vi "Imaging_Proc.vi"(5 "BioMAP file path":path=path "", 7 "Params.":variant, 8 "error in (no error)":errorcluster, 9 "Dynamic Params queue":refnum<queue>, 10 "Quit_UserEvent":refnum<user-event>, 11 "ControlQueueRef":variant) -> (0 "error out":errorcluster, 2 "Output":variant)   [LabVIEW 2013]
uses:
  Apps_static/ScanParams_SingleLine.ctl
  Files/BinaryHeader.ctl
  ControlDef/QueueRefs.ctl
  ControlDef/LaserCtrl_Method.ctl
  ControlDef/States-AToF.ctl
  <instrlib>/AnalogDiscSDKLv/VIs/DWF_CtrlQueue.ctl
  <instrlib>/AnalogDiscSDKLv/VIs/DWF_State.ctl
  <instrlib>/ESP300/Public/Data/ESP300_State.ctl
  <instrlib>/DG535/Command/DG535_States.ctl
  Hardware/BNC(QuantumComposers)/BNC_States.ctl
  Hardware/FemtoLaser(Legacy)/Laser_Status.ctl
  Hardware/DAQmx(Legacy)/DAQmx_Status.ctl
  ControlDef/Signal.ctl
  ProcessMethods/SignalAverager/ProcessStates.ctl
  Files/WriterState.ctl
  Files/Signal_Segment.ctl
  ControlDef/ProcessingMode.ctl
  Hardware/EPM2000(Legacy)/EPM2K_Status.ctl
  <instrlib>/AnalogDiscSDKLv/VIs/DWF_Signal.ctl
  ControlDef/SampleRateSelector.ctl
  DirectImaging_State.ctl
  Imaging_Params.ctl
  ProcessMethods/BioMapConversion/BioMAPWriterCoreParams.ctl
  ProcessMethods/Binning/BinType.ctl
  <vilib>/Utility/error.llb/DialogType.ctl
  <vilib>/Utility/miscctls.llb/LVRowAndColumnTypeDef.ctl
  <vilib>/picture/picture.llb/imagedata.ctl
  <userlib>/_OpenG.lib/comparison/comparison.llb/I32 Changed__ogtk.vi
  <vilib>/regexp/Match Regular Expression.xnode
  <instrlib>/ESP300/ESP300.lvlib
  <instrlib>/DG535/SRS_DG535_Lib.lvlib
  <userlib>/Utility/ErrorLog_lib.lvlib
  <instrlib>/AnalogDiscSDKLv/AnalogDiscSDKLv.lvlib
panel:
  out "POI diag.":cluster{"m/z":dbl, "Width(+/-)":dbl}[](array[cluster])
  in  "Contrast":cluster{dbl, dbl}(slide)={0.0, 255.0} scale=0.0..255.0
  in  "MaxiMass":dbl=300.0 format="%#_13g"
  in  "EnableBinning":bool
  out "Information":string
  in  "AutoScaleZ":bool
  in  "SaveImage":bool
  in  "Color Scheme":T1(ring)=enum."Rainbow"
  out "#SOL":i32
  out "#EOL":i32
  out "remaining lines":i32
  out "State":T2(ring)
  out "Line#":i32
  in  "Cancel":bool
  in  "Close/Quit":bool
  in  "Peaks of Interest":string[][](table)=[["300", "300"], ["58", ".45"], ["92", ".45"], ["114", ".45"]]
  in  "conv. coeff.":sgl=6553.0
  out "# average":i32
  in  "Start":bool
  out "ImagePreview":dbl[][](graph)
  in  "PeakOI #":i32 min=0 step=1
  out "MS (Raw)":cluster{"m/z_Array":dbl[], sgl[]}(graph)
  out "Iteration":i32
  out "Export File Path":path caption="Filename"
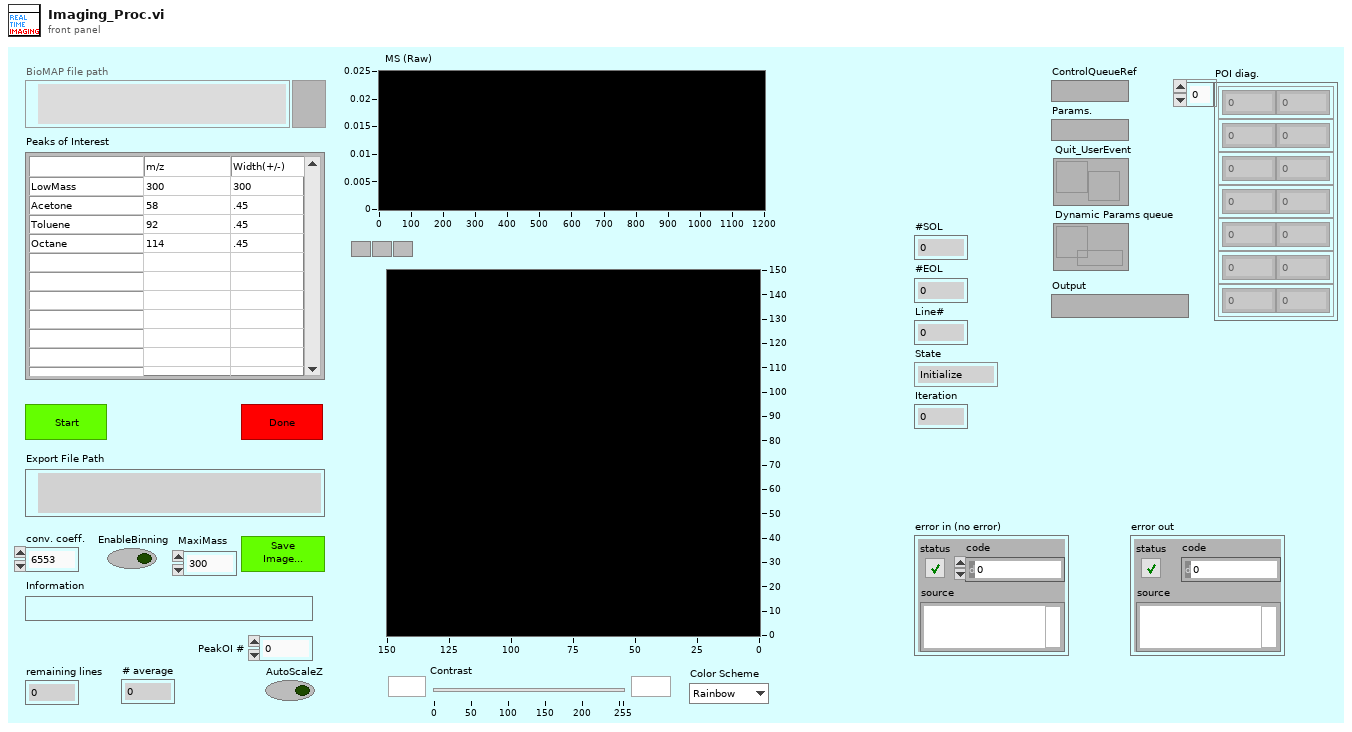
[diagram p1: front panel]
types:
  T1 = enum16{"Greyscale", "Rainbow", "Jet", "Rainbow_Wh", "Banded", "Seis", "InvertSeis", "Jaisnd", "TBD1"}
  T2 = enum16{"Initialize", "Open", "PrepScanParams", "WaitData", "Flush", "ScanResult", "CheckEndCondition", "Close", "Quit", "Refresh_Image", "Refresh_Profile", "Refresh_Spectra", "Refresh_RawSpectrum", "SaveMiddleFile", "Save_Image", "SetPeakOI"}
  T3 = cluster{"image path":path, "file refnum":refnum<file>}
  T4 = enum8{"Enabled", "Disabled", "Disabled and Grayed Out"}
  T5 = typedef "QueueRefs.ctl" = cluster{"LaserCtrlMethod":T6, "Apps":refnum<queue>, "MainDAQCoreQueue":refnum<queue>, "Micos":refnum<queue>, "ESP300":refnum<queue>, "SMC100":refnum<queue>, "SRS DG535":refnum<queue>, "BNC":refnum<queue>, "SDG_ii":refnum<queue>, "NI-USB_DAQmx":refnum<queue>, "ProcCore_CtrlQueue":refnum<queue>, "WriterCtrl":refnum<queue>, "WriterSIG":refnum<queue>, "Feedback":refnum<queue>, "EPM2000":refnum<queue>, "InfoRef":refnum<vi>, "AppsLock":T7, "ProcCore_SignalQueue":refnum<queue>}
  T6 = typedef "LaserCtrl_Method.ctl" = enum16{"SRS_DG535", "BNC", "SDG_II"}
  T7 = typedef "Semaphore RefNum" = refnum<k1>
  T8 = typedef "ProcessStates.ctl" = enum16{"Initialize", "Normal", "Display", "Write2Buffer", "CalcMzArray", "StartSave", "StopSave", "ConfigChanged", "EndOfLine", "SetFilterParams", "SetGraphsEnable", "SetAcquisitionParams", "ChangeDisplayIncrement", "ChangeRepRate", "SetWriterRef", "Quit", "StartOfLine"}
  T9 = cluster{"Average":i32, "X (Img)":i32, "Y (Img)":i32, "Spectra":sgl[]}
  T10 = typedef "BioMAPWriterCoreParams.ctl" = cluster{"File Header":T11, "mzCali.":dbl[], "m/z_Array":dbl[], "SampleRate":T12, "TrigDelay":dbl, "file refnum":refnum<file>, "file path":path, "PeakOI":cluster{"m/z":dbl, "Width(+/-)":dbl}[], "Binning":cluster{"Enable":bool, "BinType":T13, "BinWidth":dbl, "Maximum":dbl, "Minimum":dbl}}
  T11 = typedef "BinaryHeader.ctl" = cluster{"Start Position":dbl[], "StepWidth":dbl[], "Dimension":i32[], "SpecLength":i32}
  T12 = typedef "SampleRateSelector.ctl" = dbl
  T13 = typedef "BinType.ctl" = enum16{"ByTime", "ByScreen", "ByMass", "ToUnitMass"}
  T14 = typedef "Imaging_Params.ctl" = cluster{"File Header":T11, "ScanSpeed":dbl, "HighSpeed":dbl, "SampleRate":T12, "Rep.Rate (Hz)":dbl, "TrigDelay":dbl, "mzCali":dbl[], "KeepStill(ms)":u32, "SaveRaw":bool}
  T15 = typedef "DirectImaging_State.ctl" = cluster{"State":enum16{"Initialize", "Open", "PrepScanParams", "WaitData", "Flush", "ScanResult", "CheckEndCondition", "Close", "Quit", "Refresh_Image", "Refresh_Profile", "Refresh_Spectra", "Refresh_RawSpectrum", "SaveMiddleFile", "Save_Image", "SetPeakOI"}, "Para.":variant}
  T16 = cluster{"Save?":bool, "File Header":T11, "Scan#":i32, "ControlRefs":T5, "HighSpeed":dbl, "ScanSpeed":dbl, "SampleRate":T12, "mzCali.":dbl[], "TrigDelay":dbl, "InfoBarRef.":refnum<vi>}
  T17 = typedef "LVRowAndColumnTypeDef.ctl" = cluster{"Row":i32, "Column":i32}
  T18 = typedef "DialogType.ctl" = u16
  T19 = enum16{"open", "replace", "create", "open or create", "replace or create", "replace or create with confirmation"}
  T20 = cluster{"queue out":refnum<queue>, "queue out":refnum<queue>}
  T21 = typedef "Signal.ctl" = cluster{"Command":T8, "Params":variant}
  T22 = typedef "Signal_Segment.ctl" = cluster{"SampleRate":dbl, "TrigDelay":dbl, "SpecLength":dbl, "DAQ_Range":dbl, "Average#":i32, "Position":dbl[], "Spectrum":sgl[], "Calibr.":dbl[], "Pressure":dbl, "Desp_LaserEnergy":dbl, "PI_LaserEnergy":dbl, "Voltages Table":sgl[][], "ProcMode":T23, "Threshold":dbl, "Comment":string, "TickCount":dbl, "Time Stamp":timestamp}
  T23 = typedef "ProcessingMode.ctl" = enum16{"None", "Drop by Threshold", "TDC Simulate", "SetFilter"}
  T24 = typedef "ScanParams_SingleLine.ctl" = cluster{"Line Start":dbl[], "Line End":dbl[], "HighSpeed":dbl, "ScanSpeed":dbl, "KeepStill(ms)":u32, "InstruParams":dbl[]}
  T25 = typedef "imagedata.ctl" = cluster{"image type":i32, "image depth":i32, "image":u8[], "mask":u8[], "colors":u32[], "Rectangle":cluster{"left":i16, "top":i16, "right":i16, "bottom":i16}}
  T26 = cluster{"Rows Per Strip":i32, "Photometric":i32, "Compression Type":i32}
  T27 = typedef "IMAQ Image.ctl" = refnum<image>
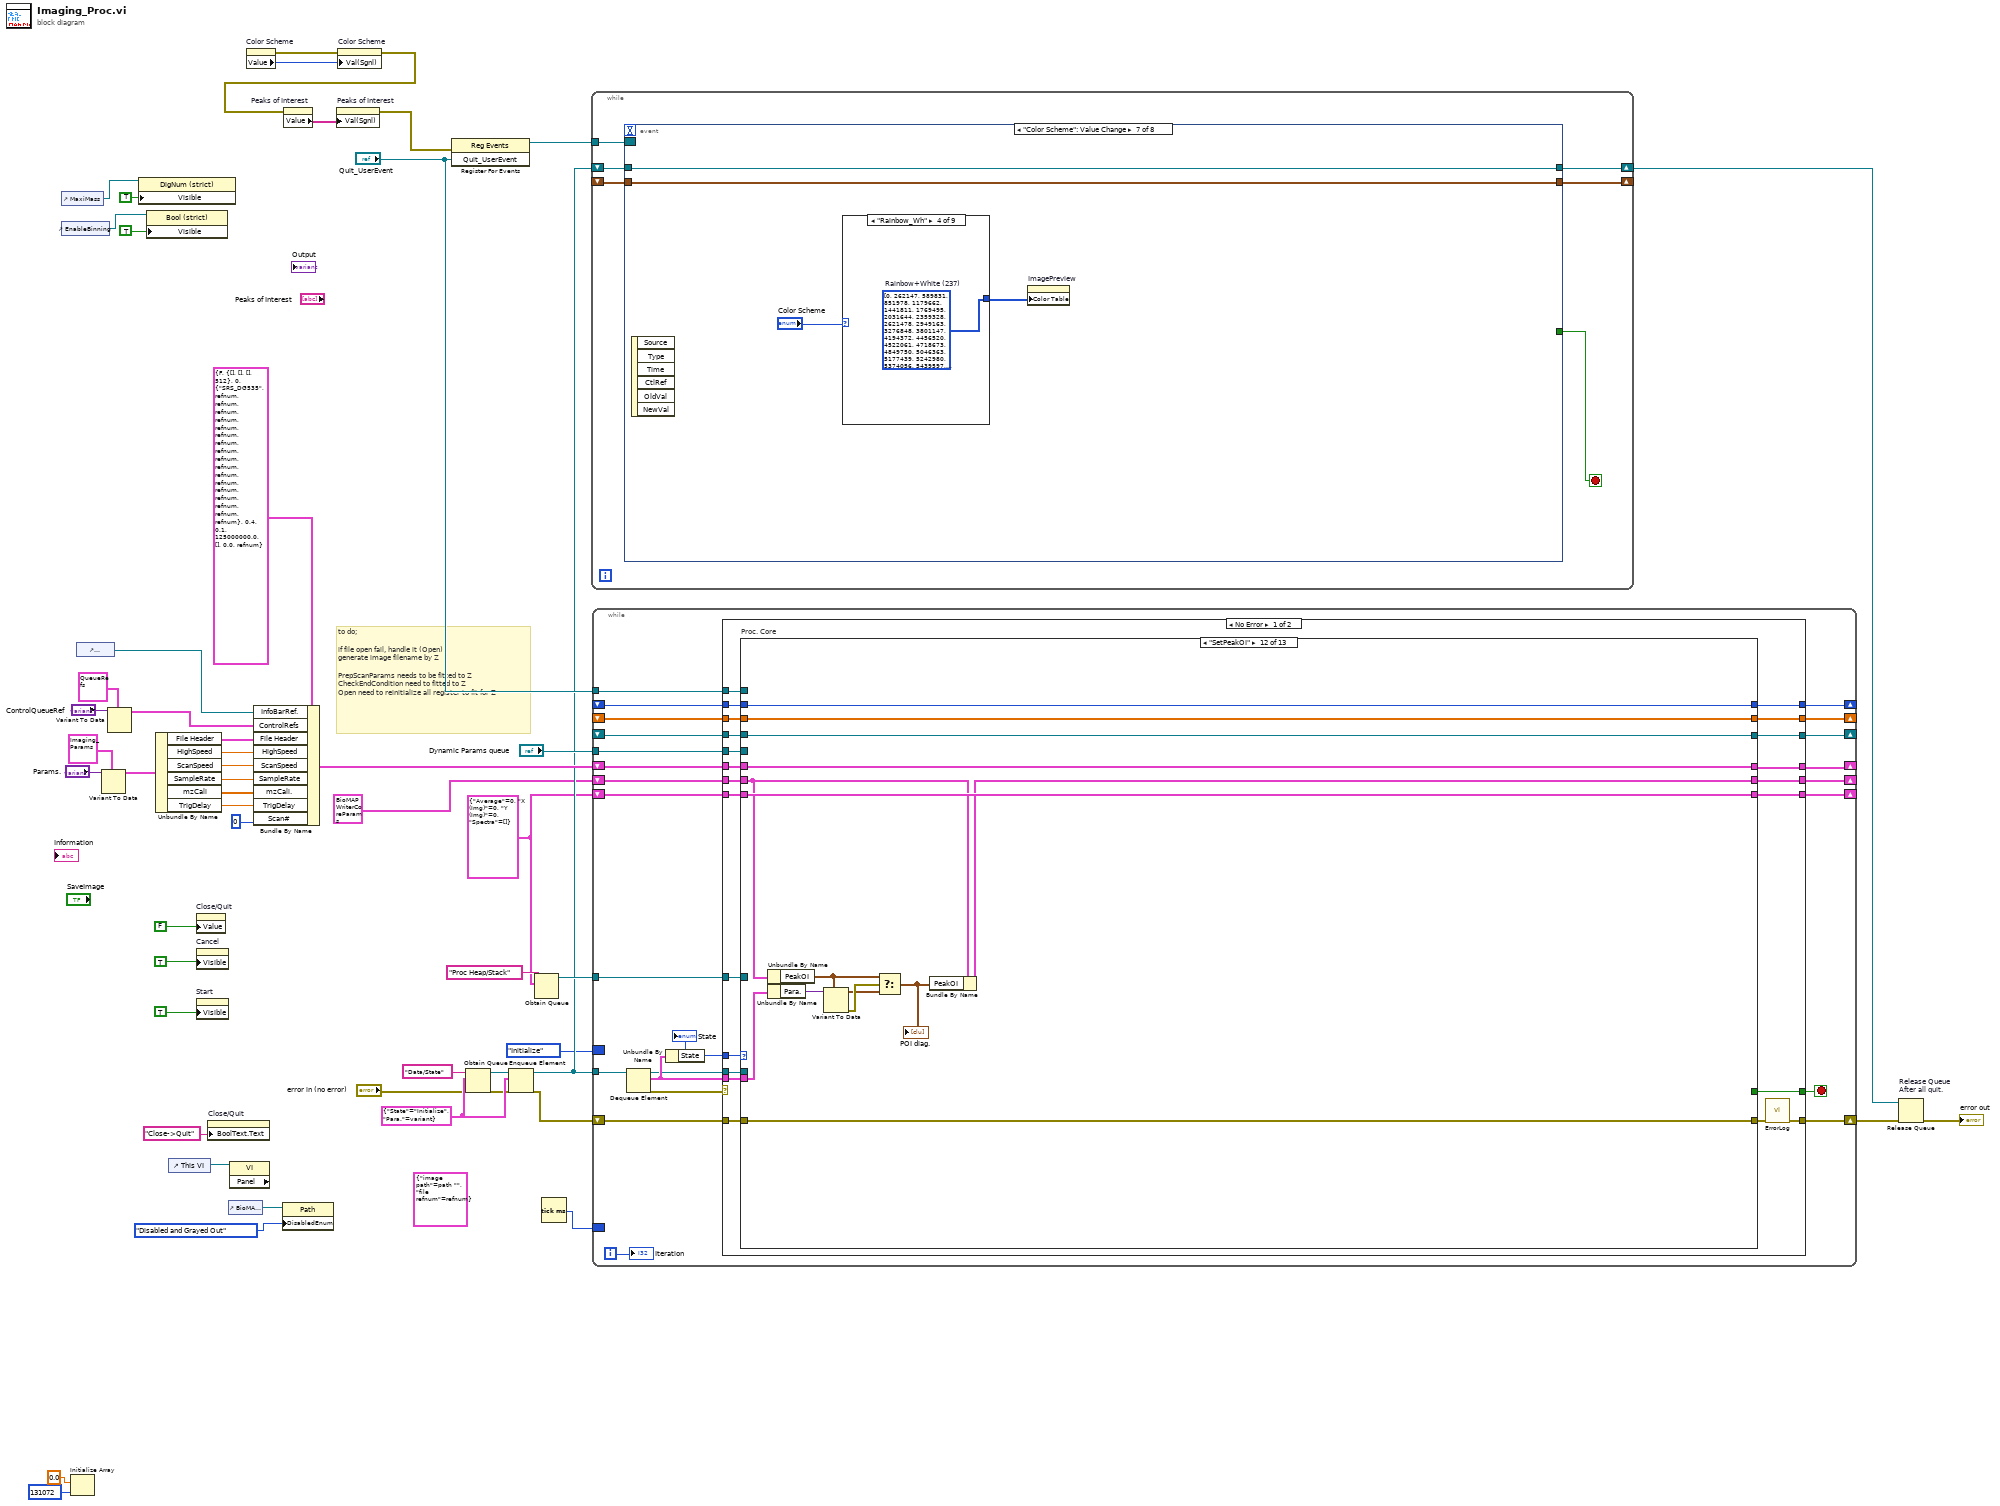
[diagram p0: block diagram]
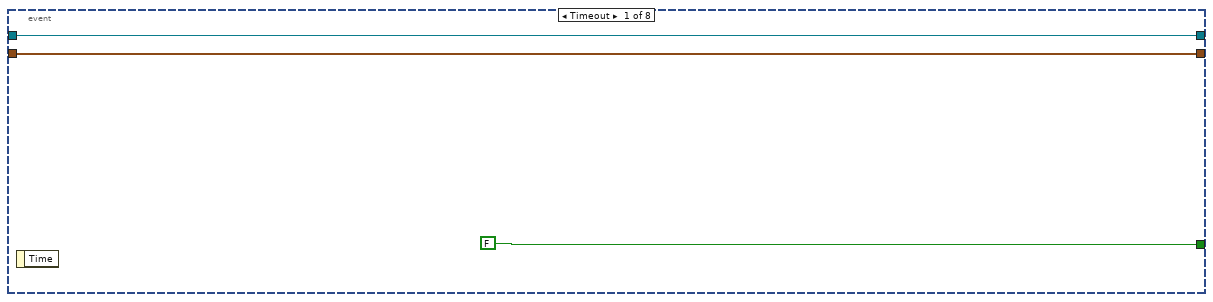
[diagram p2: hidden frame]
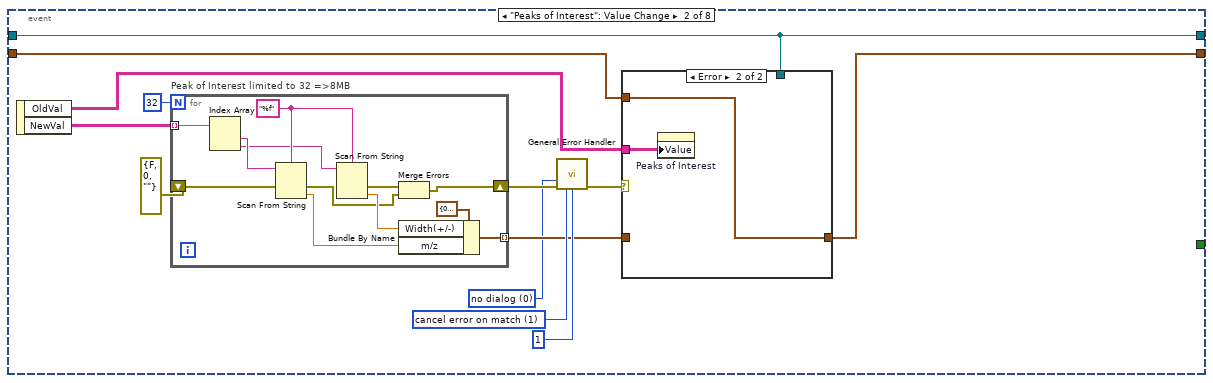
[diagram p3: hidden frame]
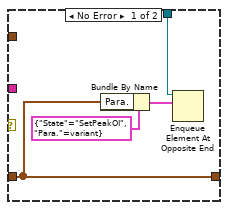
[diagram p4: hidden frame]
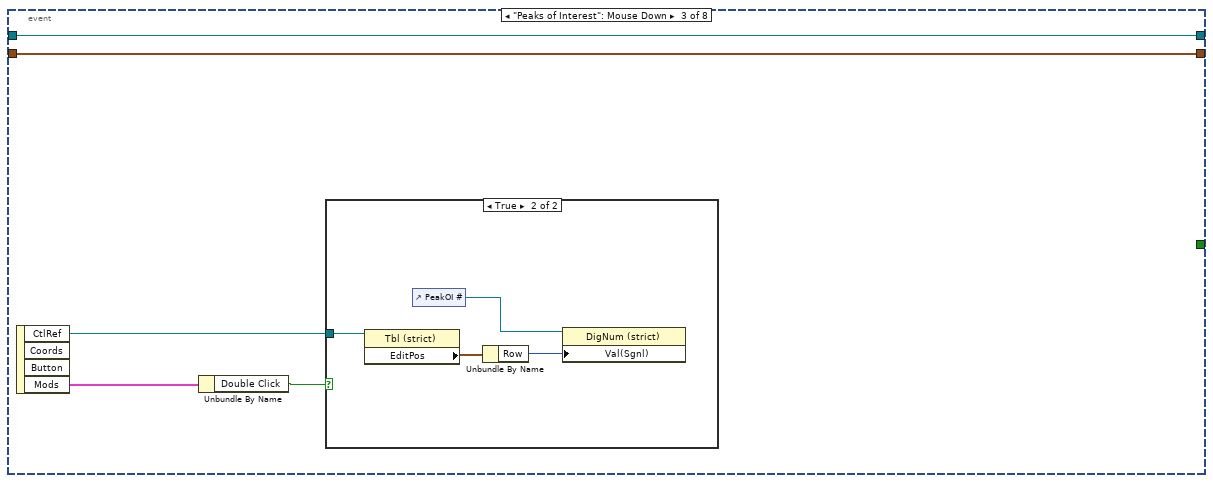
[diagram p5: hidden frame]
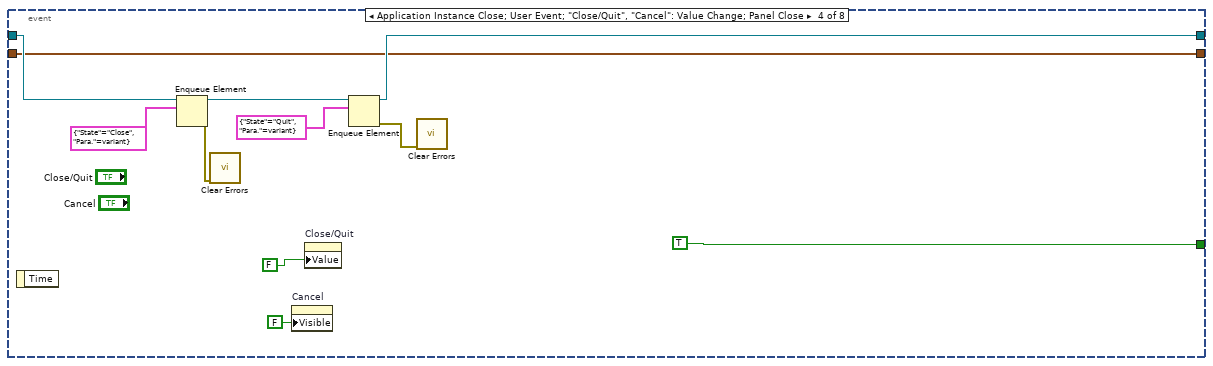
[diagram p7: hidden frame]
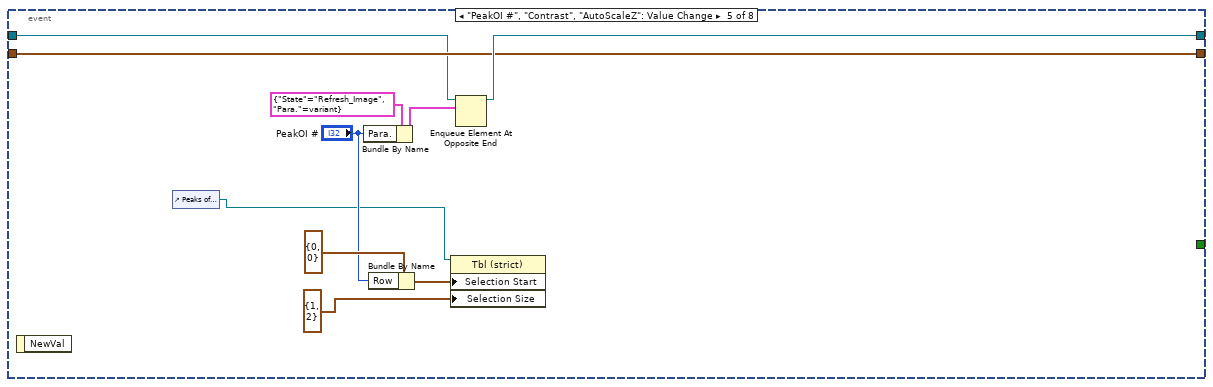
[diagram p8: hidden frame]
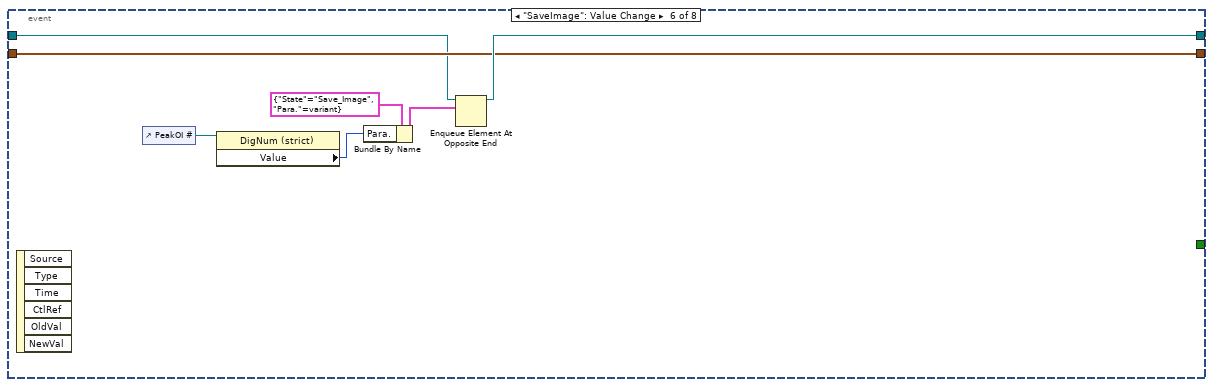
[diagram p9: hidden frame]
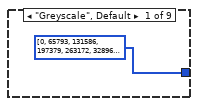
[diagram p10: hidden frame]
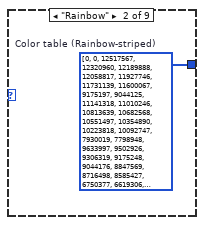
[diagram p11: hidden frame]
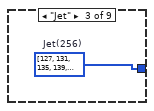
[diagram p12: hidden frame]
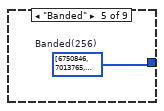
[diagram p13: hidden frame]
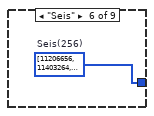
[diagram p14: hidden frame]
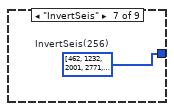
[diagram p15: hidden frame]
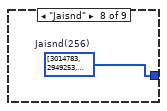
[diagram p16: hidden frame]
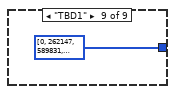
[diagram p17: hidden frame]
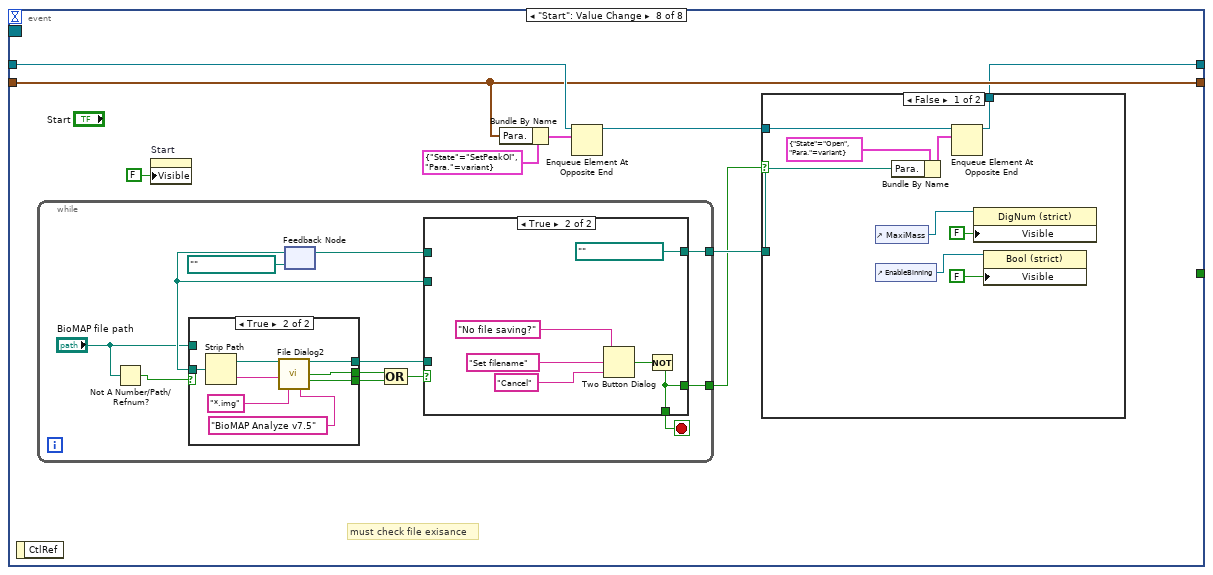
[diagram p18: hidden frame]
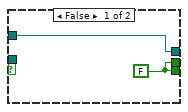
[diagram p20: hidden frame]
diagram:
  (unwired) T3 {"image path"=path "", "file refnum"=refnum} ("output cluster")
  w31 = T9 {"Average"=0, "X (Img)"=0, "Y (Img)"=0, "Spectra"=[]} ("output cluster")
  w43 = T15 {"State"=enum."Initialize", "Para."=variant}
  # "to do;\n\nif file open fail, handle it (Open)\ngenerate image filename by Z\n\nPrepScanParams needs to be fitted to Z\nCheckEndCondition need to fitted to Z\nOpen need to reinitialize all register to fit for Z"
  n1 = control-ref of="MaxiMass"() -> (w4:refnum<vi>)
  n2 = control-ref of="EnableBinning"() -> (w1:refnum<vi>)
  n3 = Initialize Array(sgl 0.0 ("element"), 131072 ("dimension size")) -> ()  [unwired: 1 out]
  n4 = control-ref of="Information"() -> (w10:refnum<vi>)
  n5 = Variant To Data(type=T14 {"File Header"={"Start Position"=[], "StepWidth"=[], "Dimension"=[], "SpecLength"=0}, "ScanSpeed"=0.0, "HighSpeed"=0.0, "SampleRate"=0.0, "Rep.Rate (Hz)"=0.0, "TrigDelay"=0.0, "mzCali"=[], "KeepStill(ms)"=0, "SaveRaw"=FALSE} ("BeamProfiling_Params"), Variant="Params.") -> (data=w38:T14)  [unwired: 1 in, 1 out]
  n6 = Variant To Data(type=T5 {"LaserCtrlMethod"=enum."SRS_DG535", "Apps"=refnum, "MainDAQCoreQueue"=refnum, "Micos"=refnum, "ESP300"=refnum, "SMC100"=refnum, "SRS DG535"=refnum, "BNC"=refnum, "SDG_ii"=refnum, "NI-USB_DAQmx"=refnum, "ProcCore_CtrlQueue"=refnum, "WriterCtrl"=refnum, "WriterSIG"=refnum, "Feedback"=refnum, "EPM2000"=refnum, "InfoRef"=refnum, "AppsLock"=refnum, "ProcCore_SignalQueue"=refnum} ("ControlRefs"), Variant="ControlQueueRef") -> (data=w18:T5)  [unwired: 1 in, 1 out]
  n7 = property class="DigNum (strict)"(reference=w4, "Visible"=TRUE) -> ()  [unwired: 1 in, 2 out]
  n8 = property class="Bool (strict)"(reference=w1, "Visible"=TRUE) -> ()  [unwired: 1 in, 2 out]
  n9 = Unbundle By Name(w38) -> ("File Header"=w37:T11, "HighSpeed"=w36:dbl, "ScanSpeed"=w35:dbl, "SampleRate"=w33:T12, "mzCali"=w24:dbl[], "TrigDelay"=w23:dbl)
  n10 = control-ref of="This VI"() -> (w22:refnum<vi>)
  n11 = property on="Close/Quit" class="Bool (strict)"("Value"=FALSE) -> ()  [unwired: 2 in, 2 out]
  n12 = property on="Cancel" class="Bool"("Visible"=TRUE) -> ()  [unwired: 2 in, 2 out]
  n13 = property on="Start" class="Bool"("Visible"=TRUE) -> ()  [unwired: 2 in, 2 out]
  n14 = property on="Close/Quit" class="Bool (strict)"("BoolText.Text"="Close->Quit" ("Boolean Text.Text")) -> ()  [unwired: 2 in, 2 out]
  n15 = control-ref of="BioMAP file path"() -> (w17:refnum<vi>)
  n16 = property class="VI" props=["Panel"](reference=w22) -> ()  [unwired: 1 in, 3 out]
  n17 = property on="Color Scheme" class="Enum (strict)"() -> (error out=w7:errorcluster, "Value"=w8:T1)  [unwired: 2 in, 1 out]
  n18 = Bundle By Name(cluster=T16 {"Save?"=FALSE, "File Header"={"Start Position"=[], "StepWidth"=[], "Dimension"=[], "SpecLength"=512}, "Scan#"=0, "ControlRefs"={"LaserCtrlMethod"=enum."SRS_DG535", "Apps"=refnum, "MainDAQCoreQueue"=refnum, "Micos"=refnum, "ESP300"=refnum, "SMC100"=refnum, "SRS DG535"=refnum, "BNC"=refnum, "SDG_ii"=refnum, "NI-USB_DAQmx"=refnum, "ProcCore_CtrlQueue"=refnum, "WriterCtrl"=refnum, "WriterSIG"=refnum, "Feedback"=refnum, "EPM2000"=refnum, "InfoRef"=refnum, "AppsLock"=refnum, "ProcCore_SignalQueue"=refnum}, "HighSpeed"=0.4, "ScanSpeed"=0.1, "SampleRate"=125000000.0, "mzCali."=[], "TrigDelay"=0.0, "InfoBarRef."=refnum} ("output cluster"), "InfoBarRef."=w10, "ControlRefs"=w18, "File Header"=w37, "HighSpeed"=w36, "ScanSpeed"=w35, "SampleRate"=w33, "mzCali."=w24, "TrigDelay"=w23, "Scan#"=0) -> (w47:T16)
  n19 = property class="Path"(reference=w17, "DisabledEnum"=T4."Disabled and Grayed Out" ("Disabled")) -> ()  [unwired: 1 in, 2 out]
  n20 = property on="Color Scheme" class="Enum (strict)"(error in=w7, "Val(Sgnl)"=w8) -> (error out=w5:errorcluster)  [unwired: 1 in, 1 out]
  n21 = property on="Peaks of Interest" class="Tbl (strict)"(error in=w5) -> ("Value"=w12:string[][])  [unwired: 1 in, 2 out]
  n22 = property on="Peaks of Interest" class="Tbl (strict)"("Val(Sgnl)"=w12) -> (error out=w6:errorcluster)  [unwired: 2 in, 1 out]
  n23 = register-events(error in=w6, "Quit_UserEvent") -> (reference out=w48:refnum<event-registration>)  [unwired: 1 in, 1 out]
  n24 = Obtain Queue(name (unnamed)="Data/State", element data type=w43, error in (no error)="error in (no error)") -> (queue out=w44:refnum<queue>, error out=w42:errorcluster)  [unwired: 2 in, 1 out]
  n25 = Enqueue Element(queue=w44, element=w43, error in (no error)=w42) -> (queue out=w40:refnum<queue>, error out=w32:errorcluster)  [unwired: 1 in, 1 out]
  n26 = Obtain Queue(name (unnamed)="Proc Heap/Stack", element data type=w31) -> (queue out=w53:refnum<queue>)  [unwired: 3 in, 2 out]
  n27 = Tick Count (ms)() -> (millisecond timer value=w30:u32)
  n28 = while {
    tunnel: w48 -> [w57]
    shift-right: [w56] -> w25
    shift-left: w40 -> [w59]
    shift-right: [w55] -> _
    shift-left: _ -> [w54]
    stop <- w58 stop-if-true
    n29 = event shown="[6] \"Color Scheme\": Value Change" {
      selector: w57 -> [_ _ _ _ _ _ _ _]
      dyn-events: _ -> [_ _ _ _ _ _ _ _]
      timeout: _ -> [_ _ _ _ _ _ _ _]
      tunnel: w59 -> [w61 w63 w98 w110 w119 w126 w134 w152]
      tunnel: [FALSE _ _ TRUE _ _ _ _] -> w58
      tunnel: [w61 w63 w98 w106 w121 w128 w134 w147] -> w56
      tunnel: [w60 w68 w94 w105 w120 w127 w131 w149] -> w55
      tunnel: w54 -> [w60 w66 w94 w105 w120 w127 w131 w149]
      event Timeout {
        n30 = event-data() -> ()  [unwired: 1 in, 1 out]
      }
      event "Peaks of Interest": Value Change {
        w64 = T18 0 items=["no dialog", "OK message", "continue or stop message", "OK message + warnings", "continue/stop + warnings"] ("type of dialog (OK msg:1)")
        w69 = 1 items=["no exception", "cancel error on match", "set error on match"] ("[exception action] (none:0)")
        n31 = event-data() -> ("OldVal"=w74:string[][], "NewVal"=w75:string[][])  [unwired: 1 in]
        n32 = for "Peak of Interest limited to 32 =>8MB" {
          N: 32 -> [_]
          tunnel: w75 -> [w87] mode=indexing
          shift-right: [w79] -> w70
          shift-left: errorcluster {"status"=FALSE, "code"=0, "source"=""} ("error IO") -> [w81]
          tunnel: [w80] -> w67 mode=indexing
          w86 = "%f" ("format string")
          n33 = Index Array(array=w87) -> (element #1=w77:string, element #2=w76:string)  [unwired: 2 in]
          n34 = Scan From String(format string=w86, input string=w77, error in=w81) -> (error out=w78:errorcluster, output 1=w83:dbl)  [unwired: 2 in, 2 out]
          n35 = Scan From String(format string=w86, input string=w76) -> (error out=w82:errorcluster, output 1=w84:dbl)  [unwired: 3 in, 2 out]
          n36 = Merge Errors(w82, w78) -> (w79:errorcluster)
          n37 = Bundle By Name(cluster=cluster{"m/z":dbl, "Width(+/-)":dbl} {"m/z"=0.0, "Width(+/-)"=0.0} ("Peak-Of-Interest"), "Width(+/-)"=w84, "m/z"=w83) -> (w80:cluster{"m/z":dbl, "Width(+/-)":dbl})
        }
        n38 = call <vilib>:"General Error Handler.vi"("type of dialog (OK msg:1)"=w64, "error in (no error)"=w70, "[exception action] (none:0)"=w69, "[exception code]"=1) -> ("error out"=w71:errorcluster)  [unwired: 7 in, 4 out]
        n39 = case shown="Error" w71 {
          tunnel: w74 -> [_ w93]
          tunnel: [w89 w92] -> w68
          tunnel: w67 -> [w89 _]
          tunnel: w66 -> [_ w92]
          tunnel: w63 -> [w88 _]
          frame No Error {
            n40 = Bundle By Name(cluster=T15 {"State"=enum."SetPeakOI", "Para."=variant} ("element"), "Para."=w89) -> (w90:T15)
            n41 = Enqueue Element At Opposite End(queue=w88, element=w90) -> ()  [unwired: 2 in, 3 out]
          }
          frame Error {
            n42 = property on="Peaks of Interest" class="Tbl (strict)"("Value"=w93) -> ()  [unwired: 2 in, 2 out]
          }
        }
      }
      event "Peaks of Interest": Mouse Down {
        n43 = event-data() -> ("CtlRef"=w95:refnum<vi>, "Mods"=w96:cluster{"Double Click":bool, "Menu Key":bool})  [unwired: 1 in, 2 out]
        n44 = Unbundle By Name(w96) -> ("Double Click"=w97:bool)
        n45 = case shown="True" w97 {
          tunnel: w95 -> [_ w101]
          frame False {
          }
          frame True {
            n46 = property class="Tbl (strict)"(reference=w101) -> ("EditPos"=w102:T17)  [unwired: 1 in, 2 out]
            n47 = control-ref of="PeakOI #"() -> (w99:refnum<vi>)
            n48 = Unbundle By Name(w102) -> ("Row"=w100:i32)
            n49 = property class="DigNum (strict)"(reference=w99, "Val(Sgnl)"=w100) -> ()  [unwired: 1 in, 2 out]
          }
        }
      }
      event Application Instance Close; User Event; "Close/Quit", "Cancel": Value Change; Panel Close {
        n50 = event-data() -> ()  [unwired: 1 in, 1 out]
        n51 = Enqueue Element(queue=w110, element=T15 {"State"=enum."Close", "Para."=variant}) -> (queue out=w111:refnum<queue>, error out=w109:errorcluster)  [unwired: 2 in, 1 out]
        n52 = call <vilib>:"Clear Errors.vi"("error in (no error)"=w109) -> ()  [unwired: 6 in, 1 out]
        n53 = property on="Cancel" class="Bool"("Visible"=FALSE) -> ()  [unwired: 2 in, 2 out]
        n54 = property on="Close/Quit" class="Bool (strict)"("Value"=FALSE) -> ()  [unwired: 2 in, 2 out]
        n55 = Enqueue Element(queue=w111, element=T15 {"State"=enum."Quit", "Para."=variant}) -> (queue out=w106:refnum<queue>, error out=w112:errorcluster)  [unwired: 2 in, 1 out]
        n56 = call <vilib>:"Clear Errors.vi"("error in (no error)"=w112) -> ()  [unwired: 6 in, 1 out]
      }
      event "PeakOI #", "Contrast", "AutoScaleZ": Value Change {
        n57 = event-data() -> ()  [unwired: 1 in, 1 out]
        n58 = control-ref of="Peaks of Interest"() -> (w114:refnum<vi>)
        n59 = Bundle By Name(cluster=T15 {"State"=enum."Refresh_Image", "Para."=variant} ("element"), "Para."="PeakOI #") -> (w122:T15)
        n60 = Bundle By Name(cluster=T17 {"Row"=0, "Column"=0} ("Selection Start"), "Row"="PeakOI #") -> (w117:T17)
        n61 = property on="Property Node" class="Tbl (strict)"(reference=w114, "Selection Start"=w117, "Selection Size"=T17 {"Row"=1, "Column"=2}) -> ()  [unwired: 1 in, 2 out]
        n62 = Enqueue Element At Opposite End(queue=w119, element=w122) -> (queue out=w121:refnum<queue>)  [unwired: 2 in, 2 out]
      }
      event "SaveImage": Value Change {
        n63 = event-data() -> ()  [unwired: 1 in, 6 out]
        n64 = control-ref of="PeakOI #"() -> (w125:refnum<vi>)
        n65 = property class="DigNum (strict)"(reference=w125) -> ("Value"=w124:i32)  [unwired: 1 in, 2 out]
        n66 = Bundle By Name(cluster=T15 {"State"=enum."Save_Image", "Para."=variant} ("element"), "Para."=w124) -> (w129:T15)
        n67 = Enqueue Element At Opposite End(queue=w126, element=w129) -> (queue out=w128:refnum<queue>)  [unwired: 2 in, 2 out]
      }
      event "Color Scheme": Value Change {
        n68 = event-data() -> ()  [unwired: 1 in, 6 out]
        n69 = case shown="\"Rainbow_Wh\"" "Color Scheme" {
          tunnel: [u32[] [0, 65793, 131586, 197379, 263172, 328965, 394758, 460551, 526344, 592137, 657930, 723723, 789516, 855309, 921102, 986895, 1052688, 1118481, 1184274, 1250067, 1315860, 1381653, 1447446, 1513239, 1579032, 1644825, 1710618, 1776411, 1842204, 1907997, 1973790, 2039583, 2105376, 2171169, 2236962, 2302755, 2368548, 2434341, 2500134, 2565927, 2631720, 2697513, 2763306, 2829099, 2894892, 2960685, 3026478, 3092271, 3158064, 3223857, 3289650, 3355443, 3421236, 3487029, 3552822, 3618615, 3684408, 3750201, 3815994, 3881787, 3947580, 4013373, 4079166, 4144959, 4210752, 4276545, 4342338, 4408131, 4473924, 4539717, 4605510, 4671303, 4737096, 4802889, 4868682, 4934475, 5000268, 5066061, 5131854, 5197647, 5263440, 5329233, 5395026, 5460819, 5526612, 5592405, 5658198, 5723991, 5789784, 5855577, 5921370, 5987163, 6052956, 6118749, 6184542, 6250335, 6316128, 6381921, 6447714, 6513507, 6579300, 6645093, 6710886, 6776679, 6842472, 6908265, 6974058, 7039851, 7105644, 7171437, 7237230, 7303023, 7368816, 7434609, 7500402, 7566195, 7631988, 7697781, 7763574, 7829367, 7895160, 7960953, 8026746, 8092539, 8158332, 8224125, 8289918, 8355711, 8421504, 8487297, 8553090, 8618883, 8684676, 8750469, 8816262, 8882055, 8947848, 9013641, 9079434, 9145227, 9211020, 9276813, 9342606, 9408399, 9474192, 9539985, 9605778, 9671571, 9737364, 9803157, 9868950, 9934743, 10000536, 10066329, 10132122, 10197915, 10263708, 10329501, 10395294, 10461087, 10526880, 10592673, 10658466, 10724259, 10790052, 10855845, 10921638, 10987431, 11053224, 11119017, 11184810, 11250603, 11316396, 11382189, 11447982, 11513775, 11579568, 11645361, 11711154, 11776947, 11842740, 11908533, 11974326, 12040119, 12105912, 12171705, 12237498, 12303291, 12369084, 12434877, 12500670, 12566463, 12632256, 12698049, 12763842, 12829635, 12895428, 12961221, 13027014, 13092807, 13158600, 13224393, 13290186, 13355979, 13421772, 13487565, 13553358, 13619151, 13684944, 13750737, 13816530, 13882323, 13948116, 14013909, 14079702, 14145495, 14211288, 14277081, 14342874, 14408667, 14474460, 14540253, 14606046, 14671839, 14737632, 14803425, 14869218, 14935011, 15000804, 15066597, 15132390, 15198183, 15263976, 15329769, 15395562, 15461355, 15527148, 15592941, 15658734, 15724527, 15790320, 15856113, 15921906, 15987699, 16053492, 16119285, 16185078, 16250871, 16316664, 16382457, 16448250, 16514043, 16579836, 16645629, 16711422, 16777215] ("Array") w136 w137 w138 w139 w140 w141 w142 u32[] [0, 262147, 589831, 851978, 1179662, 1441811, 1769495, 2031644, 2359328, 2621478, 2949163, 3276848, 3801147, 4194372, 4456520, 4522061, 4718673, 4849750, 5046363, 5177439, 5242980, 5374056, 5439597, 5505142, 5636218, 5767300, 5636232, 5701773, 5701777, 5701782, 5570714, 5505183, 5505187, 5505192, 5177521, 5111990, 5046458, 4980927, 4587720, 4456652, 4325585, 3932374, 3801306, 3604703, 3014888, 2818284, 2621681, 2359541, 2162938, 1638655, 1048831, 786687, 262399, 255, 1279, 4351, 5631, 6655, 7679, 9983, 11007, 12031, 13311, 16383, 17407, 18687, 21759, 23039, 24063, 25087, 27391, 28415, 29439, 30719, 32767, 34815, 36095, 39167, 40447, 41471, 42495, 44799, 45823, 46847, 48127, 50175, 51199, 55551, 56575, 57855, 58879, 59903, 62207, 63231, 64255, 65535, 65526, 65522, 65518, 65505, 65496, 65492, 65483, 65479, 65475, 65471, 65467, 65458, 65454, 65450, 65437, 65432, 65424, 65415, 65411, 65407, 65403, 65394, 65390, 65386, 65382, 65369, 65364, 65360, 65356, 65343, 65339, 65335, 65326, 65322, 65318, 65305, 65301, 65296, 65292, 65288, 65280, 589568, 851712, 1441536, 1703680, 1965824, 2817792, 3079936, 3407616, 3669760, 4194048, 4456192, 4783872, 5046016, 5897984, 6160128, 6422272, 7274240, 7536384, 7864064, 8126208, 8650496, 8912640, 9240320, 9502464, 10092288, 10616576, 10878720, 11730688, 11992832, 12320512, 12582656, 13106944, 13369088, 13696768, 13958912, 14548736, 14810880, 15924992, 16187136, 16449280, 16776960, 16775680, 16773632, 16772608, 16771328, 16770304, 16768256, 16766976, 16765952, 16762624, 16760576, 16759552, 16757248, 16756224, 16755200, 16753920, 16752896, 16750848, 16749568, 16748544, 16745216, 16744192, 16742144, 16739840, 16738816, 16737792, 16736512, 16734464, 16733440, 16732160, 16731136, 16727808, 16726784, 16725760, 16724736, 16721408, 16720384, 16719104, 16717056, 16716032, 16714752, 16711680, 16711680, 16711680, 16711680, 16711680, 16711680, 16711680, 16711680, 16711680, 16711680, 16711680, 16711680, 16711680, 16711680, 16711680, 16711680, 16711680, 16711680, 15527148, 15592941, 15658734, 15724527, 15790320, 15856113, 15921906, 15987699, 16053492, 16119285, 16185078, 16250871, 16316664, 16382457, 16448250, 16514043, 16579836, 16645629, 16711422, 16777215] ("appended array")] -> w132
          frame "Greyscale", Default {
          }
          frame "Rainbow" {
            w136 = u32[] [0, 0, 12517567, 12320960, 12189888, 12058817, 11927746, 11731139, 11600067, 9175197, 9044125, 11141318, 11010246, 10813639, 10682568, 10551497, 10354890, 10223818, 10092747, 7930019, 7798948, 9633997, 9502926, 9306319, 9175248, 9044176, 8847569, 8716498, 8585427, 6750377, 6619306, 8126677, 7995606, 7798999, 7667927, 7536856, 7340249, 7209178, 7078106, 5505199, 5374128, 6619357, 6488285, 6291678, 6160607, 6029536, 5832929, 5701857, 5570786, 4325557, 4194486, 5112036, 4980965, 4784358, 4653287, 4522215, 4325608, 4194537, 4063466, 3080380, 3014844, 3604716, 3408109, 3277038, 3277038, 3145966, 3014895, 2818288, 2687217, 2556145, 1900738, 1769666, 2097396, 1900789, 1769717, 1638646, 1507575, 1310968, 1179896, 1048825, 721096, 590024, 590075, 393468, 262397, 131326, 255, 1791, 3327, 4863, 5068, 6348, 9471, 11007, 12543, 14079, 15615, 17151, 18687, 20223, 17612, 18636, 25087, 26623, 28159, 29695, 31231, 32767, 34303, 35839, 29900, 31180, 40447, 41983, 43775, 45311, 46847, 48383, 49919, 51455, 42444, 43724, 56063, 57599, 59135, 60671, 62207, 63743, 65535, 65528, 52418, 52413, 65510, 65504, 65498, 65492, 65486, 65480, 65474, 65468, 52369, 52364, 65449, 65443, 65437, 65431, 65425, 65419, 65413, 65407, 52321, 52316, 65389, 65383, 65377, 65371, 65364, 65358, 65352, 65346, 52272, 52267, 65328, 65322, 65316, 65310, 65304, 65298, 65292, 65286, 52224, 314368, 851712, 1244928, 1638144, 2031360, 2424576, 2817792, 3211008, 3604224, 3197952, 3525632, 4783872, 5177088, 5635840, 6029056, 6422272, 6815488, 7208704, 7601920, 6409216, 6736896, 6736896, 8781568, 9174784, 9568000, 9961216, 10354432, 10747648, 11206400, 11599616, 9554944, 9882624, 12779264, 13172480, 13565696, 13958912, 14352128, 14745344, 15138560, 15531776, 12766208, 13093888, 16776960, 16775170, 16773637, 16771847, 16770314, 16768780, 16766991, 16765457, 13411088, 13409810, 16760601, 16758812, 16757278, 16755745, 16753955, 16752422, 16750888, 16749099, 13398052, 13396774, 16744243, 16742704, 16741166, 16739884, 16738345, 16736807, 16735269, 16733730, 13385753, 13384728, 16729371, 16727833, 16726295, 16725012, 16723474, 16721936, 16720397, 16718859, 13373959, 13372677, 16714500, 16712962, 16777215]  # Color table (Rainbow-striped)
          }
          frame "Jet" {
            w137 = u32[] [127, 131, 135, 139, 143, 147, 151, 155, 159, 163, 167, 171, 175, 179, 183, 187, 191, 195, 199, 203, 207, 211, 215, 219, 223, 227, 231, 235, 239, 243, 247, 251, 255, 1279, 2303, 3327, 4351, 5375, 6399, 7423, 8447, 9471, 10495, 11519, 12543, 13567, 14591, 15615, 16639, 17663, 18687, 19711, 20735, 21759, 22783, 23807, 24831, 25855, 26879, 27903, 28927, 29951, 30975, 31999, 33023, 34047, 35071, 36095, 37119, 38143, 39167, 40191, 41215, 42239, 43263, 44287, 45311, 46335, 47359, 48383, 49407, 50431, 51455, 52479, 53503, 54527, 55551, 56575, 57599, 58623, 59647, 60671, 61695, 62719, 63743, 64767, 131069, 393209, 655349, 917489, 1179629, 1441769, 1703909, 1966049, 2228189, 2490329, 2752469, 3014609, 3276749, 3538889, 3801029, 4063169, 4325309, 4587449, 4849589, 5111729, 5373869, 5636009, 5898149, 6160289, 6422429, 6684569, 6946709, 7208849, 7470989, 7733129, 7995269, 8257409, 8519549, 8781689, 9043829, 9305969, 9568109, 9830249, 10092389, 10354529, 10616669, 10878809, 11140949, 11403089, 11665229, 11927369, 12189509, 12451649, 12713789, 12975929, 13238069, 13500209, 13762349, 14024489, 14286629, 14548769, 14810909, 15073049, 15335189, 15597329, 15859469, 16121609, 16383749, 16645889, 16776192, 16775168, 16774144, 16773120, 16772096, 16771072, 16770048, 16769024, 16768000, 16766976, 16765952, 16764928, 16763904, 16762880, 16761856, 16760832, 16759808, 16758784, 16757760, 16756736, 16755712, 16754688, 16753664, 16752640, 16751616, 16750592, 16749568, 16748544, 16747520, 16746496, 16745472, 16744448, 16743424, 16742400, 16741376, 16740352, 16739328, 16738304, 16737280, 16736256, 16735232, 16734208, 16733184, 16732160, 16731136, 16730112, 16729088, 16728064, 16727040, 16726016, 16724992, 16723968, 16722944, 16721920, 16720896, 16719872, 16718848, 16717824, 16716800, 16715776, 16714752, 16713728, 16712704, 16711680, 16449536, 16187392, 15925248, 15663104, 15400960, 15138816, 14876672, 14614528, 14352384, 14090240, 13828096, 13565952, 13303808, 13041664, 12779520, 12517376, 12255232, 11993088, 11730944, 11468800, 11206656, 10944512, 10682368, 10420224, 10158080, 9895936, 9633792, 9371648, 9109504, 8847360, 8585216, 8323072]  # Jet(256)
          }
          frame "Rainbow_Wh" {
            w138 = u32[] [0, 262147, 589831, 851978, 1179662, 1441811, 1769495, 2031644, 2359328, 2621478, 2949163, 3276848, 3801147, 4194372, 4456520, 4522061, 4718673, 4849750, 5046363, 5177439, 5242980, 5374056, 5439597, 5505142, 5636218, 5767300, 5636232, 5701773, 5701777, 5701782, 5570714, 5505183, 5505187, 5505192, 5177521, 5111990, 5046458, 4980927, 4587720, 4456652, 4325585, 3932374, 3801306, 3604703, 3014888, 2818284, 2621681, 2359541, 2162938, 1638655, 1048831, 786687, 262399, 255, 1279, 4351, 5631, 6655, 7679, 9983, 11007, 12031, 13311, 16383, 17407, 18687, 21759, 23039, 24063, 25087, 27391, 28415, 29439, 30719, 32767, 34815, 36095, 39167, 40447, 41471, 42495, 44799, 45823, 46847, 48127, 50175, 51199, 55551, 56575, 57855, 58879, 59903, 62207, 63231, 64255, 65535, 65526, 65522, 65518, 65505, 65496, 65492, 65483, 65479, 65475, 65471, 65467, 65458, 65454, 65450, 65437, 65432, 65424, 65415, 65411, 65407, 65403, 65394, 65390, 65386, 65382, 65369, 65364, 65360, 65356, 65343, 65339, 65335, 65326, 65322, 65318, 65305, 65301, 65296, 65292, 65288, 65280, 589568, 851712, 1441536, 1703680, 1965824, 2817792, 3079936, 3407616, 3669760, 4194048, 4456192, 4783872, 5046016, 5897984, 6160128, 6422272, 7274240, 7536384, 7864064, 8126208, 8650496, 8912640, 9240320, 9502464, 10092288, 10616576, 10878720, 11730688, 11992832, 12320512, 12582656, 13106944, 13369088, 13696768, 13958912, 14548736, 14810880, 15924992, 16187136, 16449280, 16776960, 16775680, 16773632, 16772608, 16771328, 16770304, 16768256, 16766976, 16765952, 16762624, 16760576, 16759552, 16757248, 16756224, 16755200, 16753920, 16752896, 16750848, 16749568, 16748544, 16745216, 16744192, 16742144, 16739840, 16738816, 16737792, 16736512, 16734464, 16733440, 16732160, 16731136, 16727808, 16726784, 16725760, 16724736, 16721408, 16720384, 16719104, 16717056, 16716032, 16714752, 16711680, 16711680, 16711680, 16711680, 16711680, 16711680, 16711680, 16711680, 16711680, 16711680, 16711680, 16711680, 16711680, 16711680, 16711680, 16711680, 16711680, 16711680, 16777215, 16777215, 16777215, 16777215, 16777215, 16777215, 16777215, 16777215, 16777215, 16777215, 16777215, 16777215, 16777215, 16777215, 16777215, 16777215, 16777215, 16777215, 16777215, 16777215]  # Rainbow+White (237)
          }
          frame "Banded" {
            w139 = u32[] [6750846, 7013765, 7211659, 7409807, 7476371, 7411604, 7214997, 7017621, 6754453, 6490776, 6358685, 6226596, 6226092, 6226101, 6226109, 6227140, 6293961, 6296012, 6297806, 6233806, 5906635, 5512904, 4922053, 4199363, 3542212, 2950855, 2425550, 2031830, 1638622, 1376741, 1246954, 1314285, 1447407, 1975278, 2305771, 2372838, 2242272, 1783259, 1323992, 799448, 340956, 79842, 15849, 17905, 151543, 481786, 1009148, 1667324, 2193914, 2457333, 2523375, 2260968, 1801698, 1276895, 752607, 360418, 99816, 36335, 38390, 237307, 632574, 1158654, 1815550, 2275323, 2537717, 2471662, 2208487, 1683426, 1158879, 634847, 308451, 48362, 50673, 52728, 316924, 777214, 1302782, 1893373, 2352122, 2548212, 2481645, 2087398, 1628129, 1038303, 580576, 254949, 60394, 62189, 129520, 392688, 851694, 1441515, 2031078, 2423264, 2552791, 2419661, 2024898, 1499321, 974770, 516526, 190124, 60844, 62635, 129707, 458153, 982695, 1572516, 2161825, 2488475, 2552211, 2353800, 1893501, 1368177, 843623, 451166, 124759, 61010, 62797, 195401, 589383, 1113670, 1703494, 2227014, 2553410, 2551868, 2287665, 1827364, 1302294, 974603, 1040900, 1239041, 1699840, 2291200, 3013379, 3866121, 4783634, 5635611, 6355746, 6878502, 7073317, 7071521, 7004697, 6938385, 7069705, 7398403, 7858688, 8515840, 9172992, 9894916, 10550795, 11140627, 11599132, 11926051, 12055590, 11988261, 11855391, 11723032, 11788047, 11984904, 12510467, 13101824, 13759232, 14416129, 15006981, 15400460, 15728149, 15858974, 15857956, 15659558, 15395620, 15065886, 14736150, 14669582, 14800391, 15128322, 15587840, 16047616, 16441345, 16637958, 16703246, 16702743, 16570656, 16307237, 15846438, 15385379, 14924316, 14660116, 14658828, 14854661, 15182337, 15641344, 16100352, 16493826, 16690440, 16690192, 16690201, 16492833, 16163878, 15703078, 15242018, 14846235, 14647058, 14645003, 14840068, 15232513, 15690496, 16083200, 16410371, 16541193, 16541202, 16410139, 16213282, 15818789, 15292709, 14831136, 14434840, 14169616, 14166537, 14360579, 14686208, 15077888, 15404288, 15600132, 15665675, 15536665, 15342119, 15015986, 14558008, 14033211, 13507643, 13047097, 12848439, 12781367, 12911162, 13107263, 13303877, 13500748, 13501524, 13371996, 13177188, 12851050, 12393581, 11869549, 11278955, 10753384, 10293092, 9963875, 9765987, 9765220, 9764967, 9699434, 9634157, 9372526, 9111662, 8719469, 8261738]  # Banded(256)
          }
          frame "Seis" {
            w140 = u32[] [11206656, 11403264, 11599872, 11796480, 11993088, 12189696, 12386304, 12582912, 12779520, 12976128, 13172736, 13369344, 13565952, 13762560, 13959168, 14155776, 14352384, 14548992, 14745600, 14942208, 15138816, 15335424, 15532032, 15728640, 15925248, 16121856, 16318464, 16515072, 16711680, 16712448, 16713216, 16713984, 16714752, 16715520, 16716288, 16717056, 16717824, 16718592, 16719360, 16720128, 16720896, 16721664, 16722432, 16723200, 16723968, 16724736, 16725504, 16726272, 16727040, 16727808, 16728576, 16729344, 16730112, 16730880, 16731648, 16732416, 16733184, 16733952, 16734720, 16735488, 16736256, 16737024, 16737792, 16738560, 16739328, 16740096, 16740864, 16741632, 16742400, 16743168, 16743936, 16744448, 16745216, 16745984, 16746752, 16747520, 16748288, 16749056, 16749824, 16750592, 16751360, 16752128, 16752896, 16753664, 16754432, 16755200, 16755968, 16756736, 16757504, 16758272, 16759040, 16759808, 16760576, 16761344, 16762112, 16762880, 16763648, 16764416, 16765184, 16765952, 16766720, 16767488, 16768256, 16769024, 16769792, 16770560, 16771328, 16772096, 16772864, 16773632, 16774400, 16775168, 16775936, 16776704, 16776960, 16776960, 16776960, 16776960, 16776960, 16776960, 16776960, 16776960, 16776960, 16776960, 16776960, 16776960, 16776960, 16776960, 16776960, 16776960, 16776960, 16776960, 16776960, 16776960, 16776960, 16776960, 16776960, 16776960, 16776960, 16776960, 16776960, 16776960, 16645888, 16252673, 15924994, 15531779, 15138565, 14745350, 14352135, 14024456, 13631241, 13238026, 12844811, 12451596, 12123917, 11730702, 11337487, 10944272, 10551057, 10223378, 9830163, 9436948, 9043733, 8650518, 8322840, 7929625, 7536410, 7143195, 6749980, 6422301, 6029086, 5766944, 5570083, 5373222, 5176617, 4979756, 4717615, 4520753, 4324148, 4127287, 3930682, 3733821, 3471679, 3274818, 3078213, 2881352, 2684747, 2487886, 2225744, 2028883, 1832278, 1635417, 1438556, 1241950, 979553, 782948, 586087, 389482, 192620, 60784, 59509, 57979, 56704, 55173, 53642, 52367, 50836, 49305, 48030, 46499, 44968, 43694, 42163, 40888, 39357, 37826, 36551, 35020, 33489, 32214, 30684, 29409, 27878, 26347, 25072, 23541, 22010, 20735, 19965, 19195, 18426, 17912, 17142, 16372, 15603, 14833, 14319, 13549, 12780, 12010, 11240, 10726, 9957, 9187, 8417, 7647, 7134, 6364, 5594, 4824, 4055, 3541, 2771, 2001, 1232, 462]  # Seis(256)
          }
          frame "InvertSeis" {
            w141 = u32[] [462, 1232, 2001, 2771, 3541, 4055, 4824, 5594, 6364, 7134, 7647, 8417, 9187, 9957, 10726, 11240, 12010, 12780, 13549, 14319, 14833, 15603, 16372, 17142, 17912, 18426, 19195, 19965, 20735, 22010, 23541, 25072, 26347, 27878, 29409, 30684, 32214, 33489, 35020, 36551, 37826, 39357, 40888, 42163, 43694, 44968, 46499, 48030, 49305, 50836, 52367, 53642, 55173, 56704, 57979, 59509, 60784, 192620, 389482, 586087, 782948, 979553, 1241950, 1438556, 1635417, 1832278, 2028883, 2225744, 2487886, 2684747, 2881352, 3078213, 3274818, 3471679, 3733821, 3930682, 4127287, 4324148, 4520753, 4717615, 4979756, 5176617, 5373222, 5570083, 5766944, 6029086, 6422301, 6749980, 7143195, 7536410, 7929625, 8322840, 8650518, 9043733, 9436948, 9830163, 10223378, 10551057, 10944272, 11337487, 11730702, 12123917, 12451596, 12844811, 13238026, 13631241, 14024456, 14352135, 14745350, 15138565, 15531779, 15924994, 16252673, 16645888, 16776960, 16776960, 16776960, 16776960, 16776960, 16776960, 16776960, 16776960, 16776960, 16776960, 16776960, 16776960, 16776960, 16776960, 16776960, 16776960, 16776960, 16776960, 16776960, 16776960, 16776960, 16776960, 16776960, 16776960, 16776960, 16776960, 16776960, 16776960, 16776704, 16775936, 16775168, 16774400, 16773632, 16772864, 16772096, 16771328, 16770560, 16769792, 16769024, 16768256, 16767488, 16766720, 16765952, 16765184, 16764416, 16763648, 16762880, 16762112, 16761344, 16760576, 16759808, 16759040, 16758272, 16757504, 16756736, 16755968, 16755200, 16754432, 16753664, 16752896, 16752128, 16751360, 16750592, 16749824, 16749056, 16748288, 16747520, 16746752, 16745984, 16745216, 16744448, 16743936, 16743168, 16742400, 16741632, 16740864, 16740096, 16739328, 16738560, 16737792, 16737024, 16736256, 16735488, 16734720, 16733952, 16733184, 16732416, 16731648, 16730880, 16730112, 16729344, 16728576, 16727808, 16727040, 16726272, 16725504, 16724736, 16723968, 16723200, 16722432, 16721664, 16720896, 16720128, 16719360, 16718592, 16717824, 16717056, 16716288, 16715520, 16714752, 16713984, 16713216, 16712448, 16711680, 16515072, 16318464, 16121856, 15925248, 15728640, 15532032, 15335424, 15138816, 14942208, 14745600, 14548992, 14352384, 14155776, 13959168, 13762560, 13565952, 13369344, 13172736, 12976128, 12779520, 12582912, 12386304, 12189696, 11993088, 11796480, 11599872, 11403264, 11206656]  # InvertSeis(256)
          }
          frame "Jaisnd" {
            w142 = u32[] [3014783, 2949253, 2818187, 2621584, 2424982, 2228379, 2031776, 1769637, 1507497, 1245358, 917682, 655542, 327866, 190, 1218, 2757, 4041, 5580, 6863, 8402, 9941, 11480, 12763, 14301, 15840, 17378, 18916, 20198, 21736, 23274, 24556, 25837, 27375, 28656, 29938, 31219, 32500, 33781, 35062, 36343, 37368, 38649, 39673, 40698, 41723, 42747, 43772, 44796, 45821, 46589, 47613, 48381, 49406, 50174, 50942, 51710, 52478, 53502, 54270, 55038, 55806, 122110, 122878, 188926, 189695, 255999, 322303, 388607, 454911, 521215, 587519, 653823, 720127, 851966, 917499, 1048568, 1114101, 1245170, 1376239, 1441772, 1572841, 1703910, 1900515, 2031584, 2162653, 2293722, 2490327, 2621396, 2818001, 3014606, 3145676, 3342281, 3538886, 3735492, 3932097, 4194239, 4390845, 4587451, 4849593, 5046199, 5308341, 5570484, 5832626, 6029233, 6356912, 6619055, 6881199, 7143343, 7471022, 7733166, 8060847, 8388527, 8716208, 9043890, 9371571, 9764789, 10158007, 10485690, 10878908, 11337664, 11730884, 12189640, 12648397, 13172690, 13762520, 14352351, 15073256, 15990772, 16515059, 16318437, 16121818, 15990737, 15925192, 15859648, 15794105, 15794098, 15728556, 15728549, 15728543, 15794074, 15794068, 15859598, 15925129, 15925124, 15990655, 16056186, 16121717, 16252785, 16318316, 16383848, 16514916, 16580448, 16711515, 16776792, 16776276, 16775760, 16775244, 16774985, 16774469, 16773954, 16773439, 16772923, 16772408, 16771893, 16771378, 16770863, 16770093, 16769578, 16769063, 16768549, 16767778, 16767264, 16766750, 16765980, 16765465, 16764695, 16763925, 16763412, 16762642, 16761872, 16761103, 16760333, 16759564, 16758538, 16757769, 16757000, 16755975, 16755206, 16754181, 16753156, 16752131, 16751106, 16684546, 16683521, 16682497, 16681472, 16680192, 16679168, 16677888, 16676608, 16675328, 16674048, 16672768, 16671488, 16604672, 16603136, 16601856, 16600320, 16533248, 16531712, 16464640, 16463104, 16396032, 16328960, 16327168, 16260096, 16192768, 16125696, 16058368, 15991296, 15925252, 15859722, 15728657, 15663128, 15532062, 15466533, 15335467, 15204401, 15073335, 14942269, 14811203, 14680137, 14483535, 14352468, 14155865, 13959262, 13762659, 13566056, 13369452, 13172848, 12910708, 12714103, 12451962, 12189821, 11927679, 11665537, 11403394, 11075716, 10813572, 10485893, 10158212, 9830532, 9437315, 9109633, 8716415, 8323197]  # Jaisnd(256)
          }
          frame "TBD1" {
          }
        }
        n70 = property on="ImagePreview" class="IntGraph (strict)"("Color Table"=w132) -> ()  [unwired: 2 in, 2 out]
      }
      event "Start": Value Change {
        # "must check file exisance"
        n71 = event-data() -> ()  [unwired: 1 in, 1 out]
        n72 = while {
          tunnel: [w169] -> w145
          tunnel: [w165] -> w144
          stop <- w170 stop-if-true
          n73 = Not A Number/Path/Refnum?(number/path/refnum="BioMAP file path") -> (NaN/Path/Refnum?=w167:bool)
          n74 = feedback #1(path "" ("selected path")) -> (w174:path)
          n75 = case shown="True" w167 {
            tunnel: w174 -> [_ w184]
            tunnel: [w176 w183] -> w172
            tunnel: [w175 w182] -> w171
            tunnel: "BioMAP file path" -> [w176 _]
            tunnel: [w175 w177] -> w163
            frame False {
              w175 = FALSE ("cancelled")
            }
            frame True {
              n76 = Strip Path(path=w184) -> (stripped path=w179:path, name=w180:string)
              n77 = call "File Dialog2"("start path"=w179, "default name"=w180, "pattern (all files)"="*.img", "pattern label"="BioMAP Analyze v7.5") -> ("selected path"=w183:path, "exists"=w177:bool, "cancelled"=w182:bool)  [unwired: 8 in, 1 out]
            }
          }
          n78 = Compound Arithmetic op=OR(w163, w171) -> (w164:bool)
          n79 = case shown="True" w164 {
            tunnel: w172 -> [w186 _]
            tunnel: [w186 w193] -> w173
            tunnel: w174 -> [_ w193]
            tunnel: [TRUE w187] -> w170
            tunnel: [w186 path "" ("selected path")] -> w169
            tunnel: [_ w187] -> w165
            frame False {
              "Export File Path" <- w186
            }
            frame True {
              n80 = Two Button Dialog(message="No file saving?", 1:"Cancel" ("F button name (\"Cancel\")"), 2:"Set filename" ("T button name (\"OK\")")) -> (T button?=w188:bool)
              n81 = Not(x=w188) -> (.not. x?=w187:bool)
            }
          }
          n82 = feedback-in #1(w173) -> ()
        }
        n83 = property on="Start" class="Bool"("Visible"=FALSE) -> ()  [unwired: 2 in, 2 out]
        n84 = Bundle By Name(cluster=T15 {"State"=enum."SetPeakOI", "Para."=variant} ("element"), "Para."=w149) -> (w150:T15)
        n85 = Enqueue Element At Opposite End(queue=w152, element=w150) -> (queue out=w146:refnum<queue>)  [unwired: 2 in, 2 out]
        n86 = case shown="False" w144 {
          tunnel: [w161 w162] -> w147
          tunnel: w146 -> [w160 w162]
          tunnel: w145 -> [w157 _]
          frame False {
            n87 = control-ref of="MaxiMass"() -> (w153:refnum<vi>)
            n88 = control-ref of="EnableBinning"() -> (w156:refnum<vi>)
            n89 = Bundle By Name(cluster=T15 {"State"=enum."Open", "Para."=variant} ("element"), "Para."=w157) -> (w158:T15)
            n90 = Enqueue Element At Opposite End(queue=w160, element=w158) -> (queue out=w161:refnum<queue>)  [unwired: 2 in, 2 out]
            n91 = property class="DigNum (strict)"(reference=w153, "Visible"=FALSE) -> ()  [unwired: 1 in, 2 out]
            n92 = property class="Bool (strict)"(reference=w156, "Visible"=FALSE) -> ()  [unwired: 1 in, 2 out]
          }
          frame True {
          }
        }
      }
    }
  }
  n93 = while {
    shift-right: [w210] -> _
    shift-left: w47 -> [w217]
    shift-right: [w209] -> _
    shift-left: _ -> [w216]
    tunnel: w40 -> [w215]
    tunnel: w53 -> [w213]
    tunnel: "Dynamic Params queue" -> [w206]
    shift-right: [w207] -> _
    shift-left: _ -> [w205]
    shift-right: [w204] -> _
    shift-left: _ -> [w203]
    tunnel: "Quit_UserEvent" -> [w202]
    shift-right: [w200] -> w27
    shift-left: w32 -> [w201]
    shift-right: [w196] -> _
    shift-left: w31 -> [w199]
    shift-right: [w197] -> _
    shift-left: T10 {"File Header"={"Start Position"=[], "StepWidth"=[], "Dimension"=[], "SpecLength"=0}, "mzCali."=[], "m/z_Array"=[], "SampleRate"=500000000.0, "TrigDelay"=0.0, "file refnum"=refnum, "file path"=path "", "PeakOI"=[], "Binning"={"Enable"=FALSE, "BinType"=enum."ByTime", "BinWidth"=0.0, "Maximum"=0.0, "Minimum"=0.0}} ("output cluster") -> [w198]
    border: w30 -> [_]
    border: ProcessStates."Initialize" -> [_]
    i -> [w194]
    stop <- w208 stop-if-true
    n94 = Dequeue Element(queue=w215) -> (queue out=w211:refnum<queue>, element=w212:T15, error out=w214:errorcluster)  [unwired: 2 in, 1 out]
    n95 = Unbundle By Name(w212) -> ("State"=w195:T2)
    "State" <- w195
    n96 = case shown="No Error" w214 {
      tunnel: w217 -> [w239 w1093]
      tunnel: [w238 w1093] -> w210
      tunnel: w216 -> [w237 w1092]
      tunnel: [w236 w1092] -> w209
      tunnel: w213 -> [w235 _]
      tunnel: w195 -> [w234 _]
      tunnel: w212 -> [w233 _]
      tunnel: w211 -> [w232 _]
      tunnel: [w231 TRUE] -> w208
      tunnel: [w230 w1090] -> w207
      tunnel: w206 -> [w229 _]
      tunnel: w205 -> [w228 w1090]
      tunnel: [w227 w1089] -> w204
      tunnel: w203 -> [w226 w1089]
      tunnel: w202 -> [w225 _]
      tunnel: w201 -> [w224 w1088]
      tunnel: [w218 w1088] -> w200
      tunnel: w199 -> [w223 w1086]
      tunnel: w198 -> [w222 w1087]
      tunnel: [w221 w1087] -> w197
      tunnel: [w220 w1086] -> w196
      frame No Error {
        n97 = case "Proc. Core" shown="\"SetPeakOI\"" w234 {
          selector: w234 -> [_ w325 w351 _ w592 w639 _ _ _ _ _ _ _]
          tunnel: w239 -> [w255 w310 w365 w407 w569 w644 w651 w824 w829 w875 w891 w1075 w1085]
          tunnel: [w241 w332 w347 w408 w569 w644 w651 w824 w829 w875 w891 w1075 w1085] -> w238
          tunnel: [w261 0 w345 w442 w580 w636 w668 w828 w845 w874 w937 w1066 w1084] -> w236
          tunnel: w237 -> [w261 _ w345 w442 w579 w636 w668 w828 w845 w874 w937 w1066 w1084]
          tunnel: w235 -> [_ _ _ w438 w557 _ _ _ w843 _ _ _ _]
          tunnel: w233 -> [_ w286 w353 w440 w593 w640 _ _ _ w866 w930 w1074 _]
          tunnel: w232 -> [_ w326 w354 w441 w594 w641 w653 _ _ _ _ _ _]
          tunnel: [_ _ _ _ _ _ _ _ TRUE _ _ _ _] -> w231
          tunnel: [w260 w309 w349 w439 w587 w638 w665 w822 w842 w869 w933 w1067 w1083] -> w230
          tunnel: w229 -> [_ _ w356 _ _ _ _ _ w835 _ _ _ _]
          tunnel: w228 -> [w260 _ w349 w439 w588 w638 w665 w822 w842 w869 w933 w1067 w1083]
          tunnel: [w259 w321 w346 w422 w591 w637 w664 w814 w841 w873 w936 w1065 w1082] -> w227
          tunnel: w226 -> [w259 _ w346 w422 w591 w637 w664 w814 w841 w873 w936 w1065 w1082]
          tunnel: w225 -> [_ _ _ _ _ _ _ _ w840 _ _ _ _]
          tunnel: w224 -> [w258 _ w344 w437 _ w635 w663 w808 w830 w872 w935 w1076 w1081]
          tunnel: [w258 w297 w343 w437 w586 w635 w663 w808 w831 w872 w935 w1076 w1081] -> w219
          tunnel: w223 -> [w244 w313 w341 w434 w590 w633 w662 w809 w833 w870 w934 w1078 w1079]
          tunnel: w222 -> [w257 w295 w342 w409 w556 w634 w650 w810 w834 w871 w890 w1072 w1080]
          tunnel: [w256 w298 w342 w409 w556 w634 w650 w810 w834 w871 w890 w1077 w1080] -> w221
          tunnel: [w244 w313 w341 w435 w590 w633 w662 w809 w833 w870 w934 w1078 w1079] -> w220
          frame "Initialize" {
            w240 = 0  # Scan#, should not be reset to 0 in "open", for 3D imaging.
            n98 = Unbundle By Name(w255) -> ("File Header.SpecLength"=w251:i32, "File Header"=w249:T11, "mzCali."=w254:dbl[], "SampleRate"=w252:T12, "TrigDelay"=w253:dbl)
            n99 = disable-structure shown="Disabled" {
              frame Disabled {
                w262 = u32[] [0, 0, 12517567, 12320960, 12189888, 12058817, 11927746, 11731139, 11600067, 9175197, 9044125, 11141318, 11010246, 10813639, 10682568, 10551497, 10354890, 10223818, 10092747, 7930019, 7798948, 9633997, 9502926, 9306319, 9175248, 9044176, 8847569, 8716498, 8585427, 6750377, 6619306, 8126677, 7995606, 7798999, 7667927, 7536856, 7340249, 7209178, 7078106, 5505199, 5374128, 6619357, 6488285, 6291678, 6160607, 6029536, 5832929, 5701857, 5570786, 4325557, 4194486, 5112036, 4980965, 4784358, 4653287, 4522215, 4325608, 4194537, 4063466, 3080380, 3014844, 3604716, 3408109, 3277038, 3277038, 3145966, 3014895, 2818288, 2687217, 2556145, 1900738, 1769666, 2097396, 1900789, 1769717, 1638646, 1507575, 1310968, 1179896, 1048825, 721096, 590024, 590075, 393468, 262397, 131326, 255, 1791, 3327, 4863, 5068, 6348, 9471, 11007, 12543, 14079, 15615, 17151, 18687, 20223, 17612, 18636, 25087, 26623, 28159, 29695, 31231, 32767, 34303, 35839, 29900, 31180, 40447, 41983, 43775, 45311, 46847, 48383, 49919, 51455, 42444, 43724, 56063, 57599, 59135, 60671, 62207, 63743, 65535, 65528, 52418, 52413, 65510, 65504, 65498, 65492, 65486, 65480, 65474, 65468, 52369, 52364, 65449, 65443, 65437, 65431, 65425, 65419, 65413, 65407, 52321, 52316, 65389, 65383, 65377, 65371, 65364, 65358, 65352, 65346, 52272, 52267, 65328, 65322, 65316, 65310, 65304, 65298, 65292, 65286, 52224, 314368, 851712, 1244928, 1638144, 2031360, 2424576, 2817792, 3211008, 3604224, 3197952, 3525632, 4783872, 5177088, 5635840, 6029056, 6422272, 6815488, 7208704, 7601920, 6409216, 6736896, 6736896, 8781568, 9174784, 9568000, 9961216, 10354432, 10747648, 11206400, 11599616, 9554944, 9882624, 12779264, 13172480, 13565696, 13958912, 14352128, 14745344, 15138560, 15531776, 12766208, 13093888, 16776960, 16775170, 16773637, 16771847, 16770314, 16768780, 16766991, 16765457, 13411088, 13409810, 16760601, 16758812, 16757278, 16755745, 16753955, 16752422, 16750888, 16749099, 13398052, 13396774, 16744243, 16742704, 16741166, 16739884, 16738345, 16736807, 16735269, 16733730, 13385753, 13384728, 16729371, 16727833, 16726295, 16725012, 16723474, 16721936, 16720397, 16718859, 13373959, 13372677, 16714500, 16712962, 16777215]  # Color table (Rainbow-striped)
                # "Probably to be deleted"
                n100 = property on="ImagePreview" class="IntGraph (strict)"("Color Table"=w262) -> ()  [unwired: 2 in, 2 out]
              }
              frame Enabled {
              }
            }
            n101 = in-place "Compensate error in float-point number calculation" {
              n102 = in-place-cluster #2(w249) -> ("StepWidth"=w263:dbl[], "Start Position"=w268:dbl[])
              n103 = Index Array(array=w263) -> (element=w267:dbl)  [unwired: 1 in]
              n104 = Multiply(x=w267, y=0.001) -> (x*y=w265:dbl)
              n105 = in-place {
                in-place-border: w265 -> [w270]
                n106 = in-place-array #3(w268, 0) -> (w271:dbl)
                n107 = Subtract(x=w271, y=w270) -> (x-y=w272:dbl)
                n108 = in-place-array #3(w272) -> (w269:dbl[])  [unwired: 1 out]
              }
              n109 = in-place-cluster #2("StepWidth"=w263, "Start Position"=w269) -> (w248:T11)
            }
            n110 = Subtract "Gage DAQ does not always gives same length spectrum"(x=w251, y=64) -> (x-y=w242:i32)
            n111 = call "CalcMzArray.vi"("TrigDelay"=w253, "Sample Rate"=w252, "Depth"=w242, "mzCali. (a/b/c)"=w254) -> ("mzArray"=w243:dbl[])  [unwired: 7 in]
            n112 = Bundle By Name(cluster=w255, "Scan#"=w240) -> (w241:T16)
            n113 = Bundle By Name(cluster=w257, "Binning.BinType"=BinType."ByMass", "Binning.BinWidth"=0.1, "Binning.Minimum"=0.0, "File Header.SpecLength"=w242, "m/z_Array"=w243, "File Header"=w248, "mzCali."=w254, "SampleRate"=w252, "TrigDelay"=w253) -> (w256:T10)
          }
          frame "Open" {
            (unwired) T20 {"queue out"=refnum, "queue out"=refnum} ("output cluster")
            w304 = "ActionCallBack" ("name (unnamed)")
            # "Save Header + MzArray first.\nIn case of program crash, \nBioMAP v3.8+ will load partial file just fine."
            # "8192x32KB*4 = 1GB\n!! attention:\nshould be big"
            n114 = Increment(x=w325) -> (x+1=w327:T2)
            n115 = Bundle By Name(cluster=w286, "State"=w327) -> (w328:T15)
            n116 = Unbundle By Name(w286) -> ("Para."=w285:variant)
            n117 = Enqueue Element(queue=w326, element=w328) -> ()  [unwired: 2 in, 3 out]
            n118 = Variant To Data(type=path "" ("selected path"), Variant=w285) -> (data=w277:path, error out=w281:errorcluster)  [unwired: 1 in]
            n119 = Open/Create/Replace File(file path (use dialog)=w277, error in=w281, operation (0:open)=T19."create", access (0:read/write)=enum16{"read/write", "read-only", "write-only"}."write-only") -> (refnum out=w275:refnum<file>, error out=w279:errorcluster)  [unwired: 2 in, 1 out]
            n120 = Obtain Queue(max queue size (-1, unlimited)=4096, name (unnamed)="BeamProfiling_Buffer", element data type=T22 {"SampleRate"=0.0, "TrigDelay"=0.0, "SpecLength"=0.0, "DAQ_Range"=0.0, "Average#"=0, "Position"=[], "Spectrum"=[], "Calibr."=[], "Pressure"=0.0, "Desp_LaserEnergy"=0.0, "PI_LaserEnergy"=0.0, "Voltages Table"=[], "ProcMode"=enum."None", "Threshold"=0.0, "Comment"="", "TickCount"=0.0, "Time Stamp"=timestamp(0 s since 1904-01-01)} ("Signal Segment")) -> (queue out=w321:refnum<queue>, error out=w320:errorcluster)  [unwired: 2 in, 1 out]
            n121 = Obtain Queue(name (unnamed)=w304, element data type=w304) -> (queue out=w301:refnum<queue>)  [unwired: 3 in, 2 out]
            n122 = case shown="Error" w279 {
              selector: w279 -> [_ w340]
              tunnel: [_ w340] -> w278
              tunnel: w277 -> [w334 w336]
              tunnel: [w334 w336] -> w276
              tunnel: w275 -> [w333 w335]
              tunnel: [w333 w335] -> w274
              frame No Error {
              }
              frame Error {
                n123 = Two Button Dialog(message="Error when create image file.", 1:"No saving" ("F button name (\"Cancel\")"), 2:"Ignore" ("T button name (\"OK\")")) -> ()  [unwired: 1 out]
              }
            }
            n124 = Unbundle By Name(w310) -> ("ControlRefs.ProcCore_CtrlQueue"=w322:refnum<queue>)
            n125 = Bundle(cluster=T20 {"queue out"=refnum, "queue out"=refnum}, "queue out"=w321, "queue out"=w301) -> (w311:T20)
            n126 = Bundle By Name(cluster=T21 {"Command"=enum."SetWriterRef", "Params"=variant} ("element"), "Command"=ProcessStates."SetWriterRef", "Params"=w311) -> (w330:T21)
            n127 = Unbundle By Name(w295) -> ("File Header.Dimension"=w307:i32[])
            n128 = Enqueue Element "Set Data queue"(queue=w322, element=w330, error in (no error)=w320) -> (queue out=w315:refnum<queue>, error out=w303:errorcluster)  [unwired: 1 in, 1 out]
            n129 = Index Array(array=w307) -> (element #1=w306:i32, element #2=w305:i32)  [unwired: 2 in]
            n130 = Dequeue Element(queue=w301, error in (no error)=w303) -> (error out=w302:errorcluster)  [unwired: 1 in, 3 out]
            n131 = Bundle By Name(cluster=T21 {"Command"=enum."SetWriterRef", "Params"=variant} ("element"), "Command"=ProcessStates."StartSave") -> (w317:T21)
            n132 = Initialize Array "Potential Insufficient Memory Source"(sgl -1.0, w306, w305, 32 ("dimension size")) -> (w309:sgl[][][])
            n133 = Unbundle By Name(w295) -> ("Binning.BinWidth"=w291:dbl, "Binning.Minimum"=w292:dbl, "m/z_Array"=w293:dbl[], "Binning.BinType"=w294:T13)
            n134 = Enqueue Element "Start Send Data"(queue=w315, element=w317, error in (no error)=w302) -> (error out=w314:errorcluster)  [unwired: 1 in, 2 out]
            n135 = call <vilib>:"Clear Errors.vi"("error in (no error)"=w314) -> ()  [unwired: 6 in, 1 out]
            n136 = Bundle By Name(cluster=w295, "Binning.Maximum"="MaxiMass", "Binning.Enable"="EnableBinning", "file path"=w276, "file refnum"=w274) -> (w298:T10)
            n137 = call "SpectrumBinning_NoGraph.vi"("XScale.Maximum"="MaxiMass", "BinType"=w294, "BinWidth"=w291, "Enable"="EnableBinning", "Signal"=w293, "m/z Array"=w293, "XScale.Minimum"=w292) -> ("m/z Array"=w290:dbl[])  [unwired: 2 in, 2 out]
            n138 = Unbundle By Name(w278) -> ("status"=w280:bool)
            n139 = Array Size(array=w290) -> (size(s)=w289:i32)
            n140 = Bundle By Name(cluster=w298, "File Header.SpecLength"=w289, "m/z_Array"=w290) -> (w296:T10)
            n141 = Not(x=w280) -> (.not. x?=w273:bool)
            n142 = call "WriteHeader+MzArray(AnalyzeV75).vi"("error in (no error)"=w278, "ImageConvParams"=w296) -> ("error out"=w297:errorcluster)  [unwired: 9 in]
            n143 = Bundle By Name(cluster=w310, "Save?"=w273) -> (w332:T16)
          }
          frame "PrepScanParams" {
            n144 = Increment(x=w351) -> (x+1=w350:T2)
            n145 = Bundle By Name(cluster=w353, "State"=w350) -> (w352:T15)
            n146 = Unbundle By Name(w365) -> ("Scan#"=w357:i32)
            n147 = Enqueue Element(queue=w354, element=w352) -> ()  [unwired: 2 in, 3 out]
            n148 = Equal To 0?(x=w357) -> (x = 0?=w366:bool)
            n149 = case shown="False" w366 {
              tunnel: w365 -> [w378 w404]
              tunnel: [w368 w400] -> w362
              tunnel: [w372 w403] -> w361
              tunnel: [w371 w402] -> w360
              tunnel: [w370 w401] -> w359
              tunnel: w357 -> [_ w385]
              tunnel: w345 -> [_ _]
              frame True {
                w367 = 0
                # "Initial scan, stick to orignal parameter"
                n150 = Unbundle By Name(w378) -> ("HighSpeed"=w371:dbl, "ScanSpeed"=w370:dbl, "File Header"=w373:T11)
                n151 = Unbundle By Name(w373) -> ("Start Position"=w368:dbl[], "StepWidth"=w376:dbl[], "Dimension"=w377:i32[])
                n152 = Index Array(array=w376, index=w367) -> (element=w375:dbl)
                n153 = Index Array(array=w377, index=w367) -> (element=w374:i32)
                n154 = Multiply(x=w375, y=w374) -> (x*y=w369:dbl)
                n155 = in-place {
                  in-place-border: w369 -> [w380]
                  n156 = in-place-array #4(w368, w367) -> (w381:dbl)
                  n157 = Add(x=w381, y=w380) -> (x+y=w379:dbl)
                  n158 = in-place-array #4(w379) -> (w372:dbl[])  [unwired: 1 out]
                }
              }
              frame False {
                w382 = 1
                w391 = 0 ("index")
                n159 = Unbundle By Name(w404) -> ("HighSpeed"=w402:dbl, "ScanSpeed"=w401:dbl, "File Header"=w393:T11)
                n160 = Unbundle By Name(w393) -> ("Start Position"=w386:dbl[], "StepWidth"=w398:dbl[], "Dimension"=w399:i32[])
                n161 = Index Array(array=w386, index #1=w391, index #2=w382) -> (element #1=w397:dbl, element #2=w388:dbl)
                n162 = Index Array(array=w398, index #1=w391, index #2=w382) -> (element #1=w395:dbl, element #2=w390:dbl)
                n163 = Index Array(array=w399, index #1=w391, index #2=w382) -> (element #1=w394:i32, element #2=w384:i32)
                n164 = Quotient & Remainder "Circle Y #"(x=w385, y=w384) -> (x-y*floor(x/y)=w383:i32)  [unwired: 1 out]
                n165 = Multiply(x=w395, y=w394) -> (x*y=w396:dbl)
                n166 = Multiply(x=w390, y=w383) -> (x*y=w389:dbl)
                n167 = Add "X"(x=w397, y=w396) -> (x+y=w392:dbl)
                n168 = Add "Y"(x=w388, y=w389) -> (x+y=w387:dbl)
                n169 = in-place {
                  in-place-border: w392 -> [w406]
                  in-place-border: w387 -> [w405]
                  # "X"
                  # "Y"
                  n170 = in-place-array #5(w386, w382) -> ()  [unwired: 1 out]
                  n171 = in-place-array #6(w386, w391, w382) -> ()  [unwired: 2 out]
                  n172 = in-place-array #5(w405) -> (w400:dbl[])  [unwired: 1 out]
                  n173 = in-place-array #6(w406, w405) -> (w403:dbl[])  [unwired: 2 out]
                }
              }
            }
            n174 = Bundle By Name(cluster=T24 {"Line Start"=[], "Line End"=[], "HighSpeed"=0.0, "ScanSpeed"=0.0, "KeepStill(ms)"=0, "InstruParams"=[]}, "HighSpeed"=w360, "ScanSpeed"=w359, "Line Start"=w362, "Line End"=w361, "KeepStill(ms)"=u32 0 ("Wait(ms)")) -> (w355:T24)
            n175 = Increment(x=w357) -> (x+1=w364:i32)
            n176 = Enqueue Element "Send scan params"(queue=w356, element=w355) -> (error out=w348:errorcluster)  [unwired: 2 in, 2 out]
            n177 = Bundle By Name(cluster=w365, "Scan#"=w364) -> (w347:T16)
            n178 = Merge Errors(w348, w344) -> (w343:errorcluster)
            n179 = call <vilib>:"Clear Errors.vi"("error in (no error)"=w348) -> ()  [unwired: 6 in, 1 out]
          }
          frame "WaitData" {
            w429 = u32 73  # A prime number to avoid artifact
            # "Only for file conversion\nNothing to do with online conversion"
            # "Potential dead lock"
            # "Need EOF detection, \nAnd set Y Dimension to current value"
            n180 = Dequeue Element "WaitSpectra"(queue=w422) -> (element=w443:T22)  [unwired: 2 in, 3 out]
            n181 = Unbundle By Name(w443) -> ("TickCount"=w416:dbl, "Position"=w427:dbl[], "Spectrum"=w420:sgl[], "Average#"=w418:i32, "Comment"=w413:string)
            n182 = Search and Replace String(input string=w413, search string="EOF" ("y")) -> (number of replacements=w411:i32)  [unwired: 6 in, 3 out]
            n183 = String Subset(string=w413, length (rest)=2 ("length (rest)")) -> (substring=w417:string)  [unwired: 1 in]
            n184 = Type Cast(type=ProcessStates."StartOfLine", x=w417) -> (*(type *) &x=w424:T8)
            n185 = Unbundle By Name(w409) -> ("File Header.Start Position"=w425:dbl[], "File Header.StepWidth"=w426:dbl[])
            n186 = Greater Than 0?(x=w411) -> (x > 0?=w410:bool)
            n187 = Select(t=ProcessStates."Quit", s=w410, f=w424) -> (s? t:f=w415:T8)
            n188 = feedback-in #7(w415) -> ()
            n189 = feedback #7() -> (w423:T8)
            n190 = Multiply(x=w420, y=w418) -> (x*y=w419:sgl[])
            n191 = case "Average Spectra in a single pixel" shown="\"Quit\"" w415 {
              tunnel: w441 -> [w463 w480 w492 w523]
              tunnel: w438 -> [w450 w477 w490 w520]
              tunnel: w440 -> [_ _ w491 w522]
              tunnel: w434 -> [w460 w476 _ w521]
              tunnel: [_ _ _ w519] -> w435
              tunnel: [w459 w475 _ w518] -> w428
              tunnel: w419 -> [_ _ _ w505]
              tunnel: w427 -> [_ _ _ w504]
              tunnel: w426 -> [_ _ _ w503]
              tunnel: w425 -> [_ _ _ w502]
              tunnel: w423 -> [_ _ _ w499]
              tunnel: [_ _ _ w497] -> _
              tunnel: w418 -> [_ _ _ w494]
              tunnel: w416 -> [_ _ _ _]
              tunnel: [w451 w469 w486 w493] -> w408
              tunnel: w407 -> [w451 w468 w486 w493]
              frame "EndOfLine" {
                # "for debug"
                # "End of Line"
                n192 = Unbundle By Name(w460) -> ("Average"=w461:i32, "Spectra"=w462:sgl[])
                n193 = Enqueue Element At Opposite End(queue=w463, element=T15 {"State"=enum."Flush", "Para."=variant}) -> ()  [unwired: 2 in, 3 out]
                n194 = To Single Precision Float(number=w462) -> (single precision float=w458:sgl[])
                n195 = To Single Precision Float(number=w461) -> (single precision float=w457:sgl)
                n196 = Divide(x=w458, y=w457) -> (x/y=w459:sgl[])
                n197 = Bundle By Name(cluster=w460, "Average"=w461, "Spectra"=w459) -> (w456:T9)
                n198 = Enqueue Element(queue=w450, element=w456) -> ()  [unwired: 2 in, 3 out]
                n199 = feedback #8(0) -> (w453:i32)
                n200 = Increment(x=w453) -> (x+1=w452:i32)
                "#EOL" <- w452
                n201 = feedback-in #8(w452) -> ()
              }
              frame "Quit" {
                # "Does NOT handle 3D image !!"
                # "For incomplete files"
                # "End of File detected (Only for incomplete file)"
                n202 = Unbundle By Name(w476) -> ("Average"=w478:i32, "Spectra"=w479:sgl[])
                n203 = disable-structure shown="Enabled" {
                  disable-tunnel: w480 -> [w484 w485]
                  disable-tunnel: [w483 w485] -> w470
                  frame Disabled {
                    n204 = Enqueue Element At Opposite End(queue=w484, element=T15 {"State"=enum."Close", "Para."=variant}) -> (queue out=w483:refnum<queue>)  [unwired: 2 in, 2 out]
                  }
                  frame Enabled {
                  }
                }
                n205 = To Single Precision Float(number=w479) -> (single precision float=w474:sgl[])
                n206 = To Single Precision Float(number=w478) -> (single precision float=w473:sgl)
                n207 = Unbundle By Name(w468) -> ("File Header.Dimension"=w467:i32[], "Scan#"=w464:i32)
                n208 = Divide(x=w474, y=w473) -> (x/y=w475:sgl[])
                n209 = Bundle By Name(cluster=w476, "Average"=w478, "Spectra"=w475) -> (w472:T9)
                n210 = Enqueue Element(queue=w477, element=w472) -> ()  [unwired: 2 in, 3 out]
                n211 = in-place {
                  in-place-border: w464 -> [w481]
                  n212 = in-place-array #9(w467, 1) -> ()  [unwired: 1 out]
                  n213 = in-place-array #9(w481) -> (w466:i32[])  [unwired: 1 out]
                }
                n214 = Enqueue Element At Opposite End(queue=w470, element=T15 {"State"=enum."Flush", "Para."=variant}) -> ()  [unwired: 2 in, 3 out]
                n215 = Bundle By Name(cluster=w468, "File Header.Dimension"=w466) -> (w469:T16)
              }
              frame "StartOfLine" {
                # "New Line"
                n216 = Enqueue Element "Implied \"WaitData\""(queue=w492, element=w491) -> ()  [unwired: 2 in, 3 out]
                n217 = Flush Queue(queue=w490) -> ()  [unwired: 1 in, 3 out]
                n218 = feedback #10(0) -> (w488:i32)
                n219 = Increment(x=w488) -> (x+1=w487:i32)
                "#SOL" <- w487
                n220 = feedback-in #10(w487) -> ()
              }
              frame Default {
                # "Legacy"
                # "Normal Spectra"
                n221 = Index Array(array=w502) -> (element #1=w513:dbl, element #2=w514:dbl)  [unwired: 2 in]
                n222 = Index Array(array=w503) -> (element #1=w515:dbl, element #2=w516:dbl)  [unwired: 2 in]
                n223 = Index Array(array=w504) -> (element #1=w498:dbl, element #2=w517:dbl)  [unwired: 2 in]
                n224 = Enqueue Element "\"WaitData\" \nImplied"(queue=w523, element=w522) -> ()  [unwired: 2 in, 3 out]
                n225 = Subtract "Y"(x=w517, y=w514) -> (x-y=w510:dbl)
                n226 = Subtract "X"(x=w498, y=w513) -> (x-y=w511:dbl)
                n227 = Divide(x=w510, y=w516) -> (x/y=w509:dbl)
                n228 = Divide(x=w511, y=w515) -> (x/y=w512:dbl)
                n229 = Round Toward -Infinity(1:w512) -> (0:w507:dbl)
                n230 = Round Toward -Infinity(1:w509) -> (0:w508:dbl)
                n231 = To Long Integer(number=w507) -> (32bit integer=w495:i32)
                n232 = To Long Integer(number=w508) -> (32bit integer=w496:i32)
                n233 = call-poly <userlib>:"Data Changed__ogtk.vi"("I32"=w496) -> ("Changed"=w497:bool)
                n234 = Bundle By Name(cluster=T9 {"Average"=0, "X (Img)"=0, "Y (Img)"=0, "Spectra"=[]} ("output cluster"), "X (Img)"=w495, "Y (Img)"=w496, "Spectra"=w505, "Average"=w494) -> (w506:T9)
                n235 = call-poly <userlib>:"Data Changed__ogtk.vi"("I32"=w495) -> ("Changed"=w500:bool)
                n236 = case shown="True" w500 {
                  tunnel: w520 -> [_ w544]
                  tunnel: w521 -> [w528 w540]
                  tunnel: [w529 w542] -> w519
                  tunnel: w506 -> [w527 w542]
                  tunnel: [w526 w539] -> w518
                  tunnel: w499 -> [_ w537]
                  frame False {
                    # "To be averaged"
                    n237 = Unbundle By Name(w527) -> ("Spectra"=w524:sgl[], "Average"=w525:i32)
                    n238 = in-place {
                      in-place-border: w524 -> [w535]
                      in-place-border: w525 -> [w533]
                      in-place-border: [w532] -> w526
                      n239 = in-place-cluster #11(w528) -> ("Spectra"=w531:sgl[], "Average"=w530:i32)
                      n240 = Compound Arithmetic op=ADD(w531, w535) -> (w532:sgl[])
                      n241 = Compound Arithmetic op=ADD(w530, w533) -> (w534:i32)
                      n242 = in-place-cluster #11("Spectra"=w532, "Average"=w534) -> (w529:T9)
                    }
                  }
                  frame True {
                    # "First one of a pixel"
                    n243 = Unbundle By Name(w540) -> ("Average"=w541:i32, "Spectra"=w545:sgl[])
                    "# average" <- w541
                    n244 = Not Equal?(x=ProcessStates."StartOfLine", y=w537) -> (x != y?=w536:bool)
                    n245 = To Single Precision Float(number=w545) -> (single precision float=w547:sgl[])
                    n246 = To Single Precision Float(number=w541) -> (single precision float=w546:sgl)
                    n247 = Divide(x=w547, y=w546) -> (x/y=w539:sgl[])
                    n248 = Bundle By Name(cluster=w540, "Average"=w541, "Spectra"=w539) -> (w543:T9)
                    n249 = case shown="True" w536 {
                      tunnel: w544 -> [_ w549]
                      tunnel: w543 -> [_ w548]
                      frame False {
                      }
                      frame True {
                        n250 = Enqueue Element ("Push previous to stack")(queue=w549, element=w548) -> ()  [unwired: 2 in, 3 out]
                      }
                    }
                  }
                }
              }
            }
            n251 = Tick Count (ms)() -> (millisecond timer value=w430:u32)
            n252 = Less?(x=w429, y=w430) -> (x < y?=w431:bool)
            n253 = feedback #12() -> (w432:u32)
            n254 = case "raw MS refresh" shown="True" w431 {
              tunnel: w428 -> [_ w448]
              tunnel: w430 -> [_ w449]
              tunnel: [w444 w449] -> w433
              tunnel: w432 -> [w444 _]
              tunnel: w409 -> [_ w446]
              frame False {
              }
              frame True {
                n255 = Unbundle By Name(w446) -> ("m/z_Array"=w447:dbl[])
                n256 = Bundle("m/z_Array"=w447, w448) -> (→"MS (Raw)":cluster{"m/z_Array":dbl[], sgl[]})  [unwired: 1 in]
              }
            }
            n257 = feedback-in #12(w433) -> ()
          }
          frame "Flush" {
            n258 = Preview Queue Element(queue=w594, timeout in ms (-1)=0) -> (queue out=w578:refnum<queue>, element=w575:T15, timed out?=w570:bool, error out=w577:errorcluster)  [unwired: 1 in]
            n259 = Not Equal?(x=T15 {"State"=enum."Close", "Para."=variant}, y=w575) -> (x != y?=w574:cluster{"State":bool, "Para.":bool})
            n260 = Unbundle By Name(w574) -> ("State"=w573:bool)
            n261 = Or(x=w573, y=w570) -> (x .or. y?=w571:bool)
            n262 = case shown="False" w571 {
              tunnel: w593 -> [_ w630]
              tunnel: w592 -> [_ w629]
              tunnel: [w624 w628] -> w585
              tunnel: [w623 w627] -> w584
              tunnel: w578 -> [w624 w626]
              tunnel: w577 -> [w623 w625]
              frame False {
              }
              frame True {
                n263 = Increment(x=w629) -> (x+1=w631:T2)
                n264 = Bundle By Name(cluster=w630, "State"=w631) -> (w632:T15)
                n265 = Enqueue Element(queue=w626, element=w632, error in (no error)=w625) -> (queue out=w628:refnum<queue>, error out=w627:errorcluster)  [unwired: 1 in, 1 out]
              }
            }
            n266 = property on="PeakOI #" class="DigNum (strict)"() -> ("Value"=w581:i32)  [unwired: 2 in, 2 out]
            n267 = Unbundle By Name(w556) -> ("Binning.Maximum"=w561:dbl, "Binning.BinWidth"=w560:dbl, "Binning.Enable"=w553:bool, "Binning.Minimum"=w559:dbl, "m/z_Array"=w554:dbl[], "Binning.BinType"=w558:T13)
            n268 = Unbundle By Name(w569) -> ("InfoBarRef."=w568:refnum<vi>)
            n269 = Bundle By Name(cluster=T15 {"State"=enum."Refresh_Image", "Para."=variant} ("element"), "Para."=w581) -> (w582:T15)
            n270 = Enqueue Element(queue=w585, element=w582, error in (no error)=w584) -> (error out=w552:errorcluster)  [unwired: 1 in, 2 out]
            n271 = Get Queue Status(queue=w557, error in (no error)=w552) -> (queue out=w562:refnum<queue>, # elements in queue=w563:i32)  [unwired: 1 in, 6 out]
            n272 = property class="Str"(reference=w568, error in=w552, "Value"="Flushing: Don't Panic. ") -> (reference out=w567:refnum<vi>)  [unwired: 1 out]
            n273 = case "Batch Binning" shown="True" w553 {
              selector: w553 -> [_ w599]
              tunnel: w563 -> [_ w607]
              tunnel: w562 -> [w597 w606]
              tunnel: w561 -> [_ w605]
              tunnel: w560 -> [_ w604]
              tunnel: w559 -> [_ w603]
              tunnel: w558 -> [_ w602]
              tunnel: [w597 w601] -> w555
              tunnel: w554 -> [w595 w600]
              tunnel: [w596 w598] -> w550
              frame False {
                n274 = Array Size(array=w595) -> (size(s)=w596:i32)
              }
              frame True {
                n275 = for {
                  N: w607 -> [_]
                  shift-right: [w616] -> w601
                  shift-left: w606 -> [w622]
                  tunnel: w605 -> [w621]
                  tunnel: w604 -> [w620]
                  tunnel: w599 -> [w619]
                  tunnel: w603 -> [w618]
                  tunnel: w602 -> [w617]
                  tunnel: w600 -> [w611]
                  tunnel: [w608] -> w598
                  n276 = Dequeue Element(queue=w622) -> (queue out=w615:refnum<queue>, element=w614:T9)  [unwired: 2 in, 2 out]
                  n277 = Unbundle By Name(w614) -> ("Spectra"=w612:sgl[])
                  n278 = call "SpectrumBinning_NoGraph.vi"("XScale.Maximum"=w621, "BinType"=w617, "BinWidth"=w620, "Enable"=w619, "Signal"=w612, "m/z Array"=w611, "XScale.Minimum"=w618) -> ("Spectrum"=w610:dbl[], "m/z Array"=w609:dbl[])  [unwired: 2 in, 1 out]
                  n279 = Bundle By Name(cluster=w614, "Spectra"=w610) -> (w613:T9)
                  n280 = Array Size(array=w609) -> (size(s)=w608:i32)
                  n281 = Enqueue Element(queue=w615, element=w613) -> (queue out=w616:refnum<queue>)  [unwired: 2 in, 2 out]
                }
              }
            }
            n282 = Increment(x=w579) -> (x+1=w580:i32)
            n283 = Bundle By Name(cluster=w556, "File Header.SpecLength"=w550) -> (w551:T10)
            n284 = call "BioMapWriteCore.vi"("conv. coeff."="conv. coeff.", "Image in"=w588, "Y_img"=w579, "Image Params"=w551, "data buffer in"=w555) -> ("error out"=w565:errorcluster, "Image out"=w587:dbl[][][])  [unwired: 4 in, 1 out]
            n285 = call <vilib>:"General Error Handler.vi"("error in (no error)"=w565) -> ("error out"=w586:errorcluster)  [unwired: 10 in, 4 out]
            n286 = property class="Str"(reference=w567, error in=w565, "Value"="") -> ()  [unwired: 2 out]
            "Line#" <- w579
          }
          frame "ScanResult" {
            # "For comapatibility with other static subprogram, drive the loop going"
            n287 = Increment(x=w639) -> (x+1=w642:T2)
            n288 = Bundle By Name(cluster=w640, "State"=w642) -> (w643:T15)
            n289 = Enqueue Element(queue=w641, element=w643) -> ()  [unwired: 2 in, 3 out]
          }
          frame "CheckEndCondition" {
            w659 = 2  # axis:Z
            w666 = 1  # axis:Y
            # "Some bug may exist"
            # "fitted for 3D imaing, \nmay not fit for binary file conversion"
            # "Add condition:\nreader quit due to file ends"
            n290 = Unbundle By Name(w651) -> ("Scan#"=w657:i32, "File Header.Dimension"=w667:i32[])
            n291 = Index Array(array=w667, index #1=w666, index #2=w659) -> (element #1=w656:i32, element #2=w648:i32)
            n292 = Multiply(x=w656, y=w648) -> (x*y=w658:i32)
            n293 = Quotient & Remainder(x=w657, y=w656) -> (x-y*floor(x/y)=w649:i32, floor(x/y)=w647:i32)
            n294 = Subtract(x=w658, y=w657) -> (x-y=→"remaining lines":i32)
            n295 = Equal To 0? "2D_Image finished?"(x=w649) -> (x = 0?=w646:bool)
            n296 = Greater Or Equal? "3D_Image finished"(x=w647, y=w648) -> (x >= y?=w645:bool)
            n297 = case "One Image Finish" shown="True" w646 {
              tunnel: w647 -> [_ w671]
              tunnel: [T15 {"State"=enum."PrepScanParams", "Para."=variant} w681] -> w654
              tunnel: w653 -> [w669 w687]
              tunnel: [w669 w686] -> w652
              tunnel: w650 -> [_ w684]
              frame False {
                # "Continue next line scan"
              }
              frame True {
                # "If the file exist, error will be thrown out \nand will crash the expt !, proper error handling needed"
                # "to be done"
                # "A signal image finished in 3D imaging."
                n298 = Unbundle By Name(w684) -> ("file path"=w682:path)
                n299 = Enqueue Element(queue=w687, element=T15 {"State"=enum."Close", "Para."=variant}) -> (queue out=w686:refnum<queue>)  [unwired: 2 in, 2 out]
                n300 = Strip Path(path=w682) -> (stripped path=w683:path, name=w672:string)
                n301 = Format Value(string ("")="_", format string="%04d", value (0)=w671) -> (output string=w677:string)
                n302 = xnode "Match Regular Expression"("input string"=w672, "regular expression"="((_[0-9]+)?)(\\..[^.]*$)") -> ("before match"=w679:string, "submatch 3"=w674:string)  [unwired: 4 in, 6 out]
                n303 = Concatenate Strings "Append depth number"(w679, w677, w674) -> (w673:string)
                n304 = Build Path(base path=w683, name or relative path=w673) -> (appended path=w680:path)
                n305 = Bundle By Name(cluster=T15 {"State"=enum."Open", "Para."=variant}, "Para."=w680) -> (w681:T15)
              }
            }
            n306 = Select(t=T15 {"State"=enum."Close", "Para."=variant}, s=w645, f=w654) -> (s? t:f=w660:T15)
            n307 = Enqueue Element(queue=w652, element=w660) -> ()  [unwired: 2 in, 3 out]
          }
          frame "Close" {
            # "need to reset registers?\n\nNo"
            n308 = Unbundle By Name(w810) -> ("file refnum"=w811:refnum<file>)
            n309 = Close File(refnum=w811, error in=w808) -> (error out=w807:errorcluster)  [unwired: 1 out]
            n310 = call <vilib>:"Clear Errors.vi"("error in (no error)"=w807) -> ()  [unwired: 6 in, 1 out]
            n311 = Unbundle By Name(w824) -> ("ControlRefs.ProcCore_CtrlQueue"=w819:refnum<queue>, "ControlRefs.WriterSIG"=w823:refnum<queue>)
            n312 = property on="Cancel" class="Bool"("Visible"=FALSE) -> ()  [unwired: 2 in, 2 out]
            n313 = property on="Close/Quit" class="Bool (strict)"("BoolText.Text"="Done" ("Boolean Text.Text")) -> ()  [unwired: 2 in, 2 out]
            n314 = Bundle By Name(cluster=T21 {"Command"=enum."SetWriterRef", "Params"=variant} ("element"), "Command"=ProcessStates."StopSave") -> (w818:T21)
            n315 = Bundle By Name(cluster=T21 {"Command"=enum."SetWriterRef", "Params"=variant} ("element"), "Command"=ProcessStates."SetWriterRef", "Params"=w823) -> (w826:T21)
            n316 = Enqueue Element(queue=w819, element=w818) -> (queue out=w817:refnum<queue>, error out=w816:errorcluster)  [unwired: 2 in, 1 out]
            n317 = Enqueue Element(queue=w817, element=w826, error in (no error)=w816) -> (error out=w815:errorcluster)  [unwired: 1 in, 2 out]
            n318 = call <vilib>:"Clear Errors.vi"("error in (no error)"=w815) -> ()  [unwired: 6 in, 1 out]
          }
          frame "Quit" {
            n319 = disable-structure shown="Enabled" {
              disable-tunnel: w835 -> [w851 _]
              disable-tunnel: w829 -> [w847 _]
              frame Enabled {
                # "maybe not needed anymore, needed to be tested!!"
                # "Bad solution: have upper level jump out wait queue"
                n320 = Unbundle By Name(w847) -> ("HighSpeed"=w846:dbl)
                n321 = Bundle By Name(cluster=T24 {"Line Start"=[], "Line End"=[], "HighSpeed"=0.0, "ScanSpeed"=0.0, "KeepStill(ms)"=0, "InstruParams"=[]} ("element"), "HighSpeed"=w846) -> (w848:T24)
                n322 = Enqueue Element(queue=w851, element=w848) -> (error out=w849:errorcluster)  [unwired: 2 in, 2 out]
                n323 = call <vilib>:"Clear Errors.vi"("error in (no error)"=w849) -> ()  [unwired: 6 in, 1 out]
              }
              frame Disabled {
              }
            }
            n324 = Release Queue(queue=w843, error in (no error)=w830) -> (error out=w832:errorcluster)  [unwired: 1 in, 2 out]
            n325 = Generate User Event(user event=w840, event data cluster=cluster{bool} {TRUE} ("event data")) -> (user event out=w838:refnum<user-event>, error out=w837:errorcluster)  [unwired: 2 in]
            n326 = Destroy User Event(user event=w838, error in=w837) -> (error out=w836:errorcluster)
            n327 = Merge Errors(w836, w832) -> (w831:errorcluster)
          }
          frame "Refresh_Image" {
            w855 = 0.0
            # "Call command has to be push to the end not start of the queue."
            n328 = Unbundle By Name(w866) -> ("Para."=w865:variant)
            n329 = Variant To Data(type=1 ("PeakOI #"), Variant=w865) -> (data=w862:i32)  [unwired: 1 in, 1 out]
            n330 = Array Subset(array=w869, index (dim 2)=w862, length (dim 2)=1 ("length")) -> (w868:dbl[][][])  [unwired: 4 in]
            n331 = control-ref of="ImagePreview"() -> (w856:refnum<vi>)
            n332 = Array Size(array=w868) -> (size(s)=w867:i32[])
            n333 = Index Array(array=w867) -> (element #1=w861:i32, element #2=w860:i32)  [unwired: 3 in, 1 out]
            n334 = Max & Min(x=w861, y=w860) -> (max(x,y)=w859:i32)  [unwired: 1 out]
            n335 = Reshape Array(w868, w861, w860) -> (w854:dbl[][])
            n336 = property on="Fix race condition \n(autoscale related)" class="IntGraph (strict)"(reference=w856, "Value"=w854) -> (reference out=w857:refnum<vi>, error out=w858:errorcluster)  [unwired: 1 in]
            n337 = property class="IntGraph (strict)" props=["ZScale", "Maximum"](reference=w857, error in=w858) -> (reference out=w852:refnum<vi>)  [unwired: 2 out]
            n338 = case shown="True" "AutoScaleZ" {
              tunnel: w854 -> [_ w879]
              tunnel: w852 -> [_ w876]
              frame False {
              }
              frame True {
                w885 = 256.0
                n339 = Array Max & Min(array=w879) -> (max value=w888:dbl, min value=w883:dbl)  [unwired: 2 out]
                n340 = Unbundle("Contrast") -> (w886:dbl, w880:dbl)
                n341 = Subtract(x=w888, y=w883) -> (x-y=w881:dbl)
                n342 = Compound Arithmetic op=MULTIPLY(invert w885, w886, w881) -> (w884:dbl)
                n343 = Compound Arithmetic op=MULTIPLY(invert w885, w881, w880) -> (w882:dbl)
                n344 = Add(x=w882, y=w883) -> (x+y=w877:dbl)
                n345 = Add(x=w883, y=w884) -> (x+y=w878:dbl)
                n346 = property class="IntGraph (strict)"(reference=w876, "ZScale.Maximum"=w877, "ZScale.Minimum"=w878) -> ()  [unwired: 1 in, 2 out]
              }
            }
            n347 = property class="IntGraph (strict)"(reference=w852, "XScale.Minimum"=w855, "XScale.Maximum"=w859, "YScale.Minimum"=w855, "YScale.Maximum"=w859) -> ()  [unwired: 1 in, 2 out]
          }
          frame "Save_Image" {
            # "Call command has to be push to the end not start of the queue."
            n348 = control-ref of="Peaks of Interest"() -> (w899:refnum<vi>)
            n349 = Unbundle By Name(w930) -> ("Para."=w929:variant)
            n350 = property class="Tbl (strict)"(reference=w899) -> ("Value"=w898:string[][])  [unwired: 1 in, 2 out]
            n351 = Variant To Data(type=1 ("PeakOI #"), Variant=w929) -> (data=w897:i32)  [unwired: 1 in, 1 out]
            n352 = Unbundle By Name(w890) -> ("file path"=w889:path)
            n353 = Index Array(array=w898, index (row) #1=w897, index (col) #1=0 ("disabled index (col)"), index (row) #2=w897, index (col) #2=1 ("disabled index (col)")) -> (element #1=w894:string, element #2=w893:string)
            n354 = control-ref of="ImagePreview"() -> (w924:refnum<vi>)
            n355 = Strip Path(path=w889) -> (stripped path=w904:path, name=w908:string)
            n356 = Array Subset(array=w933, index (dim 2)=w897, length (dim 2)=1 ("length")) -> (w932:dbl[][][])  [unwired: 4 in]
            n357 = property class="IntGraph (strict)" props=["Color Table", "ZScale", "Maximum", "ZScale", "Minimum", "XScale", "Minimum", "XScale", "Maximum", "YScale", "Minimum", "YScale", "Maximum"](reference=w924) -> ("Color Table"=w901:u32[], "ZScale.Maximum"=w902:dbl, "ZScale.Minimum"=w903:dbl)  [unwired: 1 in, 6 out]
            n358 = xnode "Match Regular Expression"("input string"=w908, "regular expression"="(\\..[^.]*$)") -> ("before match"=w921:string)  [unwired: 4 in, 4 out]
            n359 = Format Into String(format string="_%s(+-%s)", w894, w893) -> (resulting string=w920:string)  [unwired: 2 in, 1 out]
            n360 = Array Size(array=w932) -> (size(s)=w931:i32[])
            n361 = Index Array(array=w931) -> (element #1=w926:i32, element #2=w925:i32)  [unwired: 3 in, 1 out]
            n362 = Concatenate Strings(w921, w920, ".png" ("string")) -> (w905:string)
            n363 = Reshape Array(w932, w926, w925) -> (w900:dbl[][])
            n364 = Subtract(x=w902, y=w903) -> (x-y=w914:dbl)
            n365 = Build Path(base path=w904, name or relative path=w905) -> (appended path=w906:path)
            n366 = Subtract(x=w900, y=w903) -> (x-y=w923:dbl[][])
            n367 = Divide(x=256.0 ("Img_coeff."), y=w914) -> (x/y=w916:dbl)
            n368 = Array Size(array=w923) -> (size(s)=w909:i32[])
            n369 = Compound Arithmetic op=MULTIPLY(w916, w923) -> (w917:dbl[][])
            n370 = Transpose 2D Array(2D array=w917) -> (transposed array=w918:dbl[][])
            n371 = Index Array(array=w909) -> (element #1=w911:i32, element #2=w912:i32)  [unwired: 2 in]
            n372 = Round Toward -Infinity(1:w918) -> (0:w919:dbl[][])
            n373 = Multiply(x=w911, y=w912) -> (x*y=w913:i32)
            n374 = To Unsigned Byte Integer(number=w919) -> (unsigned 8bit integer=w910:u8[][])
            n375 = disable-structure shown="Enabled" {
              disable-tunnel: w901 -> [w949 _]
              disable-tunnel: w906 -> [w948 w952]
              disable-tunnel: w910 -> [w944 w953]
              disable-tunnel: w911 -> [w942 _]
              disable-tunnel: w912 -> [w941 _]
              disable-tunnel: w913 -> [w940 _]
              frame Enabled {
                n376 = Reshape Array(w944, w940) -> (w943:u8[])
                n377 = Bundle By Name(cluster=T25 {"image type"=0, "image depth"=32, "image"=[], "mask"=[], "colors"=[], "Rectangle"={"left"=0, "top"=0, "right"=256, "bottom"=256}} ("Image Data 2"), "colors"=w949, "image type"=0, "image depth"=8, "image"=w943, "Rectangle.right"=w942, "Rectangle.bottom"=w941) -> (w939:T25)
                n378 = call <vilib>:"Write PNG File.vi"("image data"=w939, "path to PNG file"=w948) -> ("error out"=w938:errorcluster)  [unwired: 8 in, 1 out]
                n379 = call <vilib>:"Clear Errors.vi"("error in (no error)"=w938) -> ()  [unwired: 6 in, 1 out]
              }
              frame Disabled {
                n380 = call "IMAQ ArrayToImage"("Image Pixels (U8)"=w953) -> ("Image Out"=w951:T27)  [unwired: 9 in, 1 out]
                n381 = call-poly "IMAQ Write File 2"("TIFF Options"=T26 {"Rows Per Strip"=0, "Photometric"=1, "Compression Type"=3}, "File Path"=w952, "Image"=w951) -> ()  [unwired: 7 in, 2 out]
              }
            }
          }
          frame "SetPeakOI" {
            n382 = Unbundle By Name(w1072) -> ("PeakOI"=w1068:cluster{"m/z":dbl, "Width(+/-)":dbl}[])
            n383 = Unbundle By Name(w1074) -> ("Para."=w1073:variant)
            n384 = Variant To Data(type=w1068, Variant=w1073) -> (data=w1070:cluster{"m/z":dbl, "Width(+/-)":dbl}[], error out=w1071:errorcluster)  [unwired: 1 in]
            n385 = Select(t=w1068, s=w1071, f=w1070) -> (s? t:f=w1069:cluster{"m/z":dbl, "Width(+/-)":dbl}[])
            "POI diag." <- w1069
            n386 = Bundle By Name(cluster=w1072, "PeakOI"=w1069) -> (w1077:T10)
          }
          frame Default {
          }
        }
        n387 = call <userlib>:"ErrorLog.vi"("error in (no error)"=w219) -> ("error out"=w218:errorcluster)  [unwired: 10 in]
      }
      frame Error {
      }
    }
    "Iteration" <- w194
  }
  n388 = Release Queue "Release Queue\nAfter all quit."(queue=w25, error in (no error)=w27) -> (error out=→"error out":errorcluster)  [unwired: 1 in, 2 out]
